vi "CreateNewProperty.vi"(5 "Physical Channels Array":string[](array[string]), 6 "JSON Text In":string, 7 "Properties Array":string[](array[string]), 8 "error IO":errorcluster, 9 "User Input":T12, 10 "Position Index":T1, 11 "Data":T2) -> (0 "error out":errorcluster, 2 "JSON Text Out":string, 3 "Data Out":T2)   [LabVIEW 2017]
uses:
  Ctrl/UserInput.ctl
  Ctrl/Data.ctl
  Ctrl/Caps.ctl
  Ctrl/Property.ctl
  Ctrl/PhysicalChannel.ctl
  Ctrl/Register.ctl
  Ctrl/Bitfield.ctl
  Ctrl/Scale.ctl
  Ctrl/ScaleType.ctl
  Ctrl/Enum.ctl
  Ctrl/EnumValue.ctl
  a49f2b7a-a89a-493e-b672-83a64a1dc848.vi
  b7239d0f-a886-4cdc-b9e9-eaf961555556.vi
  9a8c8dea-2cdf-4e02-b2f8-f2feb6ef9a15.vi
  ea6883c3-21c4-4fa9-9e68-a5003e32a3fd.vi
  c685517d-3b86-4edc-b318-7cf002de9467.vi
  83024576-e123-423a-a292-784f9ca3acef.vi
  5d470e54-f309-4a2d-b700-b5160160c7a0.vi
  2d628e2e-8e77-4fc1-a05a-5f0eb3d140a3.vi
  3a93f355-f44d-43be-885c-c8174923e2df.vi
  69acab33-e041-4299-87fe-07d24066ef73.vi
  f5ba869a-ac95-4e4c-86ff-dad057e8b940.vi
  a7fe37d0-f046-4b52-bd49-58630115636d.vi
  21b13566-51c8-4b08-b7be-3dce8c990445.vi
  f01481eb-adc2-4292-a7dc-d6c3eaadea6e.vi
  0f458bcc-7b61-44ae-a900-99c499cd9c3b.vi
  c10375a5-0795-48be-8fad-3286e309e908.vi
  5c14b599-8786-4955-9b75-2db17ef63de3.vi
  6e15b919-6c59-4ef2-a7c0-28ece143eb9f.vi
  7c4f7e53-dbd1-4e39-b078-caddc5d3bffd.vi
  11ea50df-9018-48f0-836e-47b654efc2ff.vi
  0e1caf04-e2e9-4b70-9720-e1a210467dd4.vi
  d58aa79e-fb29-4d7b-acaf-7e78ee01c68a.vi
  24b307f7-ae9b-4334-a273-07ddeeb49d19.vi
  49acb1fb-1d23-4d16-8d65-d3f60ea831e1.vi
  6c8c26da-812b-44f4-8a47-b287122740a3.vi
  6e470968-faeb-473e-94d4-9f473792bd2a.vi
  576f94e5-2af0-4523-a9f0-3304e6cbc8c1.vi
  7c2c566b-f820-4e15-b4ed-1f65cd12d5f0.vi
  0f012f77-c120-4dc7-a671-207e81cb5f49.vi
  25a589fe-9d62-4a78-be02-6bcfab6bb56e.vi
  f3b9646e-74a6-4e13-b3dc-42ccebcfd1e8.vi
  d27e821d-89cf-46bb-b5e1-9624ca9468fb.vi
  6a42c134-5544-4b97-a994-3a894c6fd8c5.vi
  628c06dd-8667-4172-93bf-cd1d4ad4abe0.vi
  4fb511c2-f303-4d71-abd1-b379f02bfd88.vi
  45fd9c47-b19a-4360-9f3e-2172322a7f8b.vi
  755fc430-c706-4afd-be3d-980f95401532.vi
  0e9b9207-256e-4707-b51c-b6ca433831fa.vi
  99d4434d-72ea-4ca1-92e2-3e4fa824596b.vi
  f10b79d4-fc05-4857-ad0d-b3836f64004d.vi
  7132fcb4-bd99-438f-a692-8292e7484c4f.vi
  cca9a672-75e7-4021-816c-68aa3c6a6872.vi
  ecd3546a-508f-424b-98fa-eb27a157b20d.vi
  0c9dfa0a-ec9d-420a-8a56-6a5b97d1e641.vi
  ccdac7b3-f8f0-4fd4-822c-79269ee8a063.vi
  3a771616-e512-457e-808b-110273b57013.vi
  d688189c-f4c5-4b6f-aec2-5bfb8a1bf2cd.vi
  ac0dcac6-9883-45e7-93cd-88fffc2866e0.vi
  3376c375-25a1-4c34-bd38-a19c28cb765e.vi
  7a403b02-5ffc-42e7-baa3-b7a4eeba28ce.vi
  01b9138b-76a2-4359-acf3-d9de97d059d9.vi
  a141bb58-9ba5-441b-868f-21200b55c099.vi
  80822c65-4f16-4974-bc2c-80759235b62b.vi
  6f6ebfe9-c60c-414d-8b12-ba3bdeeaba59.vi
  a52452e6-86e2-4211-9ca9-267b4c83b3c9.vi
  dbfa2163-7e2d-4f30-9237-4ef7c0592618.vi
  91ed7ecc-eecc-4599-94e1-676a613ecbb1.vi
  ae2bc896-6ce6-4903-bc84-87fefb09e09c.vi
  113ba1ce-32d2-48ad-819e-36eabf9c747b.vi
  4d7999a1-46fe-4a82-956d-b90eb1783e73.vi
  fd5b9c13-e0cd-4f6e-a59d-9b48d1913b00.vi
  bf6c18ca-27a2-471c-8ef5-1202f5916418.vi
  8917d4d8-2e68-438d-a95d-91d892a45299.vi
  37f20183-cbb6-408d-bc9b-499ea9cc8cf1.vi
  17a8dd43-fc52-448d-8aba-334e99b77679.vi
  8211e012-3519-4404-b0b3-339e76ea4bc1.vi
  509dba11-f6b1-40d4-b7e2-c91f78e09c4c.vi
  3b6dfc74-68ce-41c5-8a3c-09f3ccd4e9e6.vi
  556964bf-9fb0-437c-b57b-6005a56280ca.vi
  c644abda-56b7-4dd7-8add-f8f48cdb8744.vi
  9f73811a-95bf-4eb4-a8fa-f38c92d15f78.vi
  bb4007d4-f8f0-4bc5-9028-5f1cf2c35148.vi
  4f7d9488-ab40-4515-a693-da524a43faec.vi
  eddbc0d9-62dd-400d-aae9-2a28a5c77658.vi
  f57e54e9-0c83-4c4f-85ea-985bd06e531a.vi
  6f79dc5f-b950-4598-84a2-cd13e182a849.vi
  61c115c5-33ef-4a3e-bc4e-0e2805e03db5.vi
  4019a736-0945-4c3d-9530-64ae120c8d82.vi
  fc220763-ec92-4a82-8c98-1888f306469b.vi
  81716be8-6f03-4c12-be78-44b8fbb8dac1.vi
  b447dfd2-34a3-4ef0-b1a0-0449a08cdddb.vi
  0c062650-fd43-4944-b945-f8cbdc6d9a08.vi
  bc4388ac-6fed-49ed-999e-9d9af0d36177.vi
  213fb9c5-0553-47a7-8513-261bde567b61.vi
  45dea8f4-95f3-403e-9396-3338e63b5c58.vi
  198f9814-5678-407e-905c-3dffdfeb1b1a.vi
  0b3e7f97-d846-4561-b743-4d2b63a05b0c.vi
  2ce1d167-041f-4eb0-a5ff-a6bbcfc02b33.vi
  d4f37732-829b-439f-949d-15773a71446b.vi
  c2cabc7c-6f3f-4e97-9c76-69ff8817e041.vi
  a0bcf8de-4f7f-4748-830e-4ca73a3cdba5.vi
  108ef926-3dca-4005-a0d1-c4fff904fb71.vi
  decae038-41de-45d0-9a85-a35aff0e32d8.vi
  232f2805-0da1-4bd2-964f-a5a57d1a0789.vi
  b481430d-8ad2-4f6e-8535-813648ab6332.vi
  30ebd30d-697e-41d4-a062-6538e9b0372d.vi
  3e2a4e09-f947-4d87-9f6b-36e026663a87.vi
  4de69aee-0985-453e-b62a-95ac3040a333.vi
  a82c2a40-5500-42ec-81fe-51a317ee7e6a.vi
  4ea25b15-c434-4186-b702-6004432441e7.vi
  1f846b06-a524-4db4-a3bc-67689fb64464.vi
  8cc0f9d5-1403-42f5-8db9-98bc4be2fcad.vi
  e01775d1-2ca2-49e0-b186-643bd2c40956.vi
  203d3e81-1240-40e6-b528-fe3fc3fb6b71.vi
  b90cfbf0-b34a-4f7c-a92c-1bf1608e7875.vi
  17010cc0-3e9d-4f94-9fb8-6f8c3e52e337.vi
  31c470be-9090-43e5-9e9c-e90aeaef58ff.vi
  65070d91-edea-43b9-8fa4-4e2d47d23c2a.vi
  223cc870-c1bd-4fed-9a4e-cb6bbe7d487d.vi
  231ecd50-a15c-4ed1-a0c9-2424d186b4de.vi
  36281ff1-d9a9-4575-bd1c-3efb6e2311e5.vi
  624e145d-2cd7-4bd9-b329-75a63af49bab.vi
  cfc68e07-b182-4d06-a56e-000b2c92bce0.vi
  0a8ea711-960b-4203-93a6-dad2a0ce5ccf.vi
  27813dee-b6cf-4adb-b65a-f979060e7e79.vi
  1f1b6db9-9b07-4b01-9a35-2055f5be4eb1.vi
  ace04026-a7e6-4f2f-b899-111909789ab4.vi
  37535dc1-fec1-4151-9bd0-9935b704efa5.vi
  db3b4f8a-2deb-4574-ad41-4f9ae64a690f.vi
  6e899c75-a155-4662-bc59-3d9896a22a99.vi
  f9819b1f-b189-4309-8c14-53bc3d75f35f.vi
  6878b97e-9808-4441-b6cb-f4989035cf89.vi
  40b71344-1fb3-4cdd-a6ad-9b0b64e136ec.vi
  9c3c6458-e941-4b27-8d55-2b4a0fd28597.vi
  39623eaf-85e6-4175-8452-6887610aa769.vi
  1149246f-1cb2-4460-baf6-518fc77c3398.vi
  94badf7b-9ba4-4923-94d3-547b74146f8e.vi
  ffb6c1ad-0599-4325-8e09-657e99a7831d.vi
  51fd1ea7-ce8f-4a70-a74f-9fc830ed3e6b.vi
  de89801e-8830-4ce5-860e-6e3e2d97c53c.vi
  455b00cc-8d48-4a28-be52-9894321e9b13.vi
  9e4596ea-b512-429e-ae0e-35bad6f11e4a.vi
  d6d440e2-9f68-4db2-b22d-75274f54af10.vi
  1256f0d8-c1ca-45fc-a187-c743900cc4a2.vi
  9439dccc-9f4c-481b-bf63-cbedd9744780.vi
  1f2e0b96-ad1d-4f53-bf6b-c3e13ad15049.vi
  4cd03f52-d737-4399-b5f9-45d06f489655.vi
  14ebd26c-c7b1-4e24-86d1-22f775b8f9ab.vi
  8a9c42ea-46d3-4fe9-9435-a8b3a4a2dbd4.vi
  3a6543c7-dfa5-4b63-b6d3-167b518bbb5e.vi
  5a92ceff-b602-480b-bb39-7b08cb863a45.vi
  d378d0bf-cb50-4329-b507-76bc9876ca06.vi
  7e87eee9-c7ed-45a5-bcca-739a3caf24b9.vi
  f2f04b58-7349-4c1d-a7d6-26891e21feea.vi
  bf4bca74-9d66-4959-9a8b-143b177785cd.vi
  04733de7-f337-4faf-8c84-b7833aa6f2cb.vi
  74f378fe-b6f6-4528-9979-942041c20273.vi
  c32d4527-d702-4456-8891-4932f3849ab6.vi
  74301831-9c69-485b-8e5c-16671aac40f0.vi
  32197667-d662-404d-af3b-3c9461875803.vi
  26d8f128-faf4-4dc7-be93-989510b637ce.vi
  f34d1c9c-ef35-4bff-872b-d236ed75701e.vi
  9c27fe3a-8c23-4b01-b34b-ef9b2563181d.vi
  a6395615-55d0-428c-9b5d-c0b31a22a7cf.vi
  f2764ccd-c2d5-4c9f-af8e-47687746aee1.vi
  e5379eb7-e7bb-42e7-910b-1b038f3940f8.vi
  a0e0f5c1-ff2b-49b7-a7b9-a60d0cd9baa7.vi
  a0b0d031-bf61-4b01-9fca-99c15f00df1f.vi
  54d28dfd-e1e7-45d6-aa43-71dfc314fd28.vi
  ab9abbc4-570d-4bb5-bc1a-691eeb63bc1d.vi
  d1ce7e24-64f3-4c43-ab40-66c03b4f9e3e.vi
  b237b2f1-2f83-437a-9cea-1bce77fd5025.vi
  044d47e4-0514-4989-8b3e-8a398604f3d7.vi
  c63cd178-caa2-4b18-8318-2349136bf0e1.vi
  4b639117-fa7a-4c0e-8ad7-bca49a2943c3.vi
  8267567e-f780-4e05-b009-d0c9ce0abba4.vi
  1625688c-520d-43a3-ab9a-e66d702972f2.vi
  44449f3f-58ce-45d9-97d0-2b38db85702a.vi
  f909daa1-f824-43b3-83b3-b8b77778ee66.vi
  a97c2141-69b1-4da5-94ca-ebac57d47087.vi
  b0e5809b-780b-4791-a098-08ecc8fea483.vi
  3022a1d8-e834-49f8-aa3d-1b2c8a074b58.vi
  a74e2ca7-2cff-4482-b120-7da61f7f9ad3.vi
  e2416475-e97a-4f09-a291-685253a7cfe7.vi
  313abf92-0b2c-41a6-89ad-da4ba565ce18.vi
  37aa6e6a-6e49-48fc-97e0-4a9a28f52783.vi
  42e813b3-8dc3-471a-9ba1-21131290105b.vi
  6f02c78c-2bb0-4da4-870c-847981bce678.vi
  006840be-01be-4ebd-9b8f-ea77a6ba57aa.vi
  83ec3a63-defe-4e3b-a6ed-e0f6b07438b7.vi
  76608141-6b6b-44ec-b072-9a8bd16893bc.vi
  661c9a8c-c5b5-406e-a622-3d4232183939.vi
  448871fc-56c7-4969-ae73-d107eae8dd61.vi
  67a8e6fe-4925-4bd0-bf84-9d9d2ff2a511.vi
  e0e6f61b-f592-4636-85da-145c07327336.vi
  05b159be-fb2d-4452-84c3-9ba3097d799d.vi
  66a5adf1-5026-465b-8117-59515cd5681b.vi
  89332561-ea55-4d6a-8c47-78ecf90b24dc.vi
  42cf89a1-8e03-4f53-8d52-799e9435a61c.vi
  96527726-a160-4a48-adef-fe795eb6a5ca.vi
  36013bd7-b93e-491b-a104-af11587fd964.vi
  f1628db2-2072-415f-964c-f240b5113352.vi
  6395648c-62af-41db-b829-02cd2fba18d1.vi
  0d4c42cd-1dc5-4f20-868b-863dbe6493db.vi
  454f590e-240f-4e40-8cf2-0be346249117.vi
  eca76937-d954-4f66-b29c-5125c898f574.vi
  ee8ef92e-b5c6-4b6c-9e99-f238648b3acd.vi
  ab44ab14-7959-48f0-b172-dac530811317.vi
  fe65aa24-0d15-4b88-8a81-a6b00e8cc108.vi
  47278b13-07ad-44b4-92ee-55cb8c7775f7.vi
  32afd39a-e2cc-43d6-8b91-cc3721be6205.vi
  72a5a9e2-8cc7-4781-b6ce-fe396b598b40.vi
  aa930b89-a957-4a40-aea5-f072bec8f2e0.vi
  ae0460c2-7f2e-440b-b89e-9afba5751a8a.vi
  d2cfe406-efaa-4813-911a-e8cc1010b633.vi
  53ced5e1-6cfb-4c56-ae99-55efe528f378.vi
  2e78f98a-ab78-448d-8ebd-4acd63531133.vi
  88442ee8-73f3-4212-ac74-ab778edeacb7.vi
  1332a019-3d0f-4c16-8ae1-7ee48909245a.vi
  df3c917c-2193-40a5-ba35-6d5d70650e51.vi
  edce4bd0-27e9-42af-8081-06bf6614b3f1.vi
  a8ec8fbb-1ef4-4c47-b821-8822cada8249.vi
  <vilib>/JDP Science/JSONtext/String Subset.vi
  <vilib>/JDP Science/JSONtext/Variant to JSON Text.vi
  <vilib>/JDP Science/JSONtext/Parsing/Parse Full Path or Item Name.vi
  <vilib>/JDP Science/JSONtext/Offset/Find Item Locations by Path.vi
  <vilib>/JDP Science/JSONtext/JSONtext.lvlib
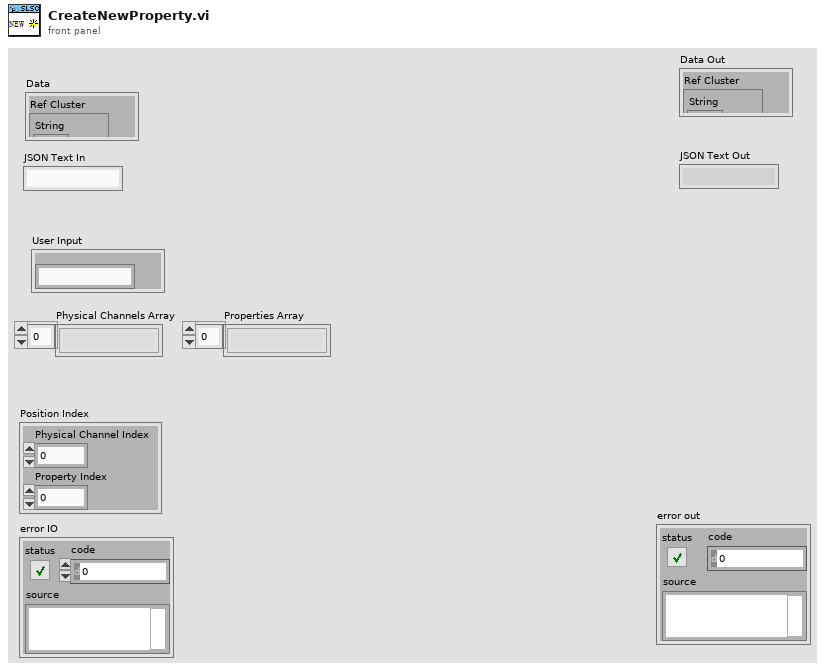
[diagram p1: front panel]
types:
  T1 = cluster{"Physical Channel Index":i32, "Property Index":i32}
  T2 = typedef "Data.ctl" = cluster{"Ref Cluster":cluster{"String":refnum<vi>, "U8":refnum<vi>, "I8":refnum<vi>, "U32":refnum<vi>, "I32":refnum<vi>, "U64":refnum<vi>, "I64":refnum<vi>, "Ring":refnum<vi>, "DBL":refnum<vi>, "Add":refnum<vi>, "Remove":refnum<vi>, "Property tree":refnum<vi>, "confirm":refnum<vi>}, "JSON Text":string, "Original JSON Text":string, "Caps":T3, "SLSC Output Tree":cluster{"Left Cell String":string, "Child Text":string[], "Child Tag":string, "Item Indent":i32, "Child Only?":bool, "Glyph Index":i32, "offline value":variant}[], "Ref Index and Control Type":cluster{"index":i32, "Datatype":string}, "Selected Type and name":cluster{"Selected Type":enum16{"Property", "Physical Channel", "Other"}, "Selected Property Name":string}, "Update whole Tree?":bool}
  T3 = typedef "Caps.ctl" = cluster{"properties":T4[], "physical channels":T5[], "registers":T6[], "scales":T8[], "enums":T10[], "productName":string}
  T4 = typedef "Property.ctl" = cluster{"name":string, "bitfield":string, "value":variant, "dataType":string, "min":variant, "max":variant, "scale":string, "access":string}
  T5 = typedef "PhysicalChannel.ctl" = cluster{"name":string, "properties":T4[]}
  T6 = typedef "Register.ctl" = cluster{"name":string, "address":i32, "size":i32, "bitfields":T7[], "initialValue":variant, "connectedProperties":string[]}
  T7 = typedef "Bitfield.ctl" = cluster{"name":string, "offset":i32, "size":i32, "signed":bool}
  T8 = typedef "Scale.ctl" = cluster{"name":string, "type":T9, "params":variant}
  T9 = typedef "ScaleType.ctl" = enum16{"NoScale", "Table", "Polynomial", "Linear"}
  T10 = typedef "Enum.ctl" = cluster{"name":string, "values":T11[]}
  T11 = typedef "EnumValue.ctl" = cluster{"name":string, "value":i32}
  T12 = typedef "UserInput.ctl" = cluster{"NewPropertyParameter":cluster{"Name":string, "DataType":enum16{"String", "Double", "U64", "I64", "U32", "I32", "Bool"}, "Bitfield":u16, "Access":u16, "Description":string, "Documentation":string, "OK Button":bool, "Scale method":u16, "Write a Register?":bool, "Write a Range?":bool, "Value_Cluster":cluster{"DBL":dbl, "Ring":u16, "I64":i64, "U64":u64, "I32":i32, "U32":u32, "I8":i8, "U8":u8, "String":string}}, "Min_Max_Cluster":cluster{"Min(Double)":dbl, "Max(Double)":dbl, "Min(U64)":u64, "Max(U64)":u64, "Min(I64)":i64, "Max(I64)":i64, "Min(U32)":u32, "Max(U32)":u32, "Min(I32)":i32, "Max(I32)":i32}, "Scale method":string, "Access":string, "Bitfield":string}
  T13 = enum16{"String", "Double", "U64", "I64", "U32", "I32", "Bool"}
  T14 = cluster{"DBL":dbl, "Ring":u16, "I64":i64, "U64":u64, "I32":i32, "U32":u32, "I8":i8, "U8":u8, "String":string}
  T15 = cluster{"Min(Double)":dbl, "Max(Double)":dbl, "Min(U64)":u64, "Max(U64)":u64, "Min(I64)":i64, "Max(I64)":i64, "Min(U32)":u32, "Max(U32)":u32, "Min(I32)":i32, "Max(I32)":i32}
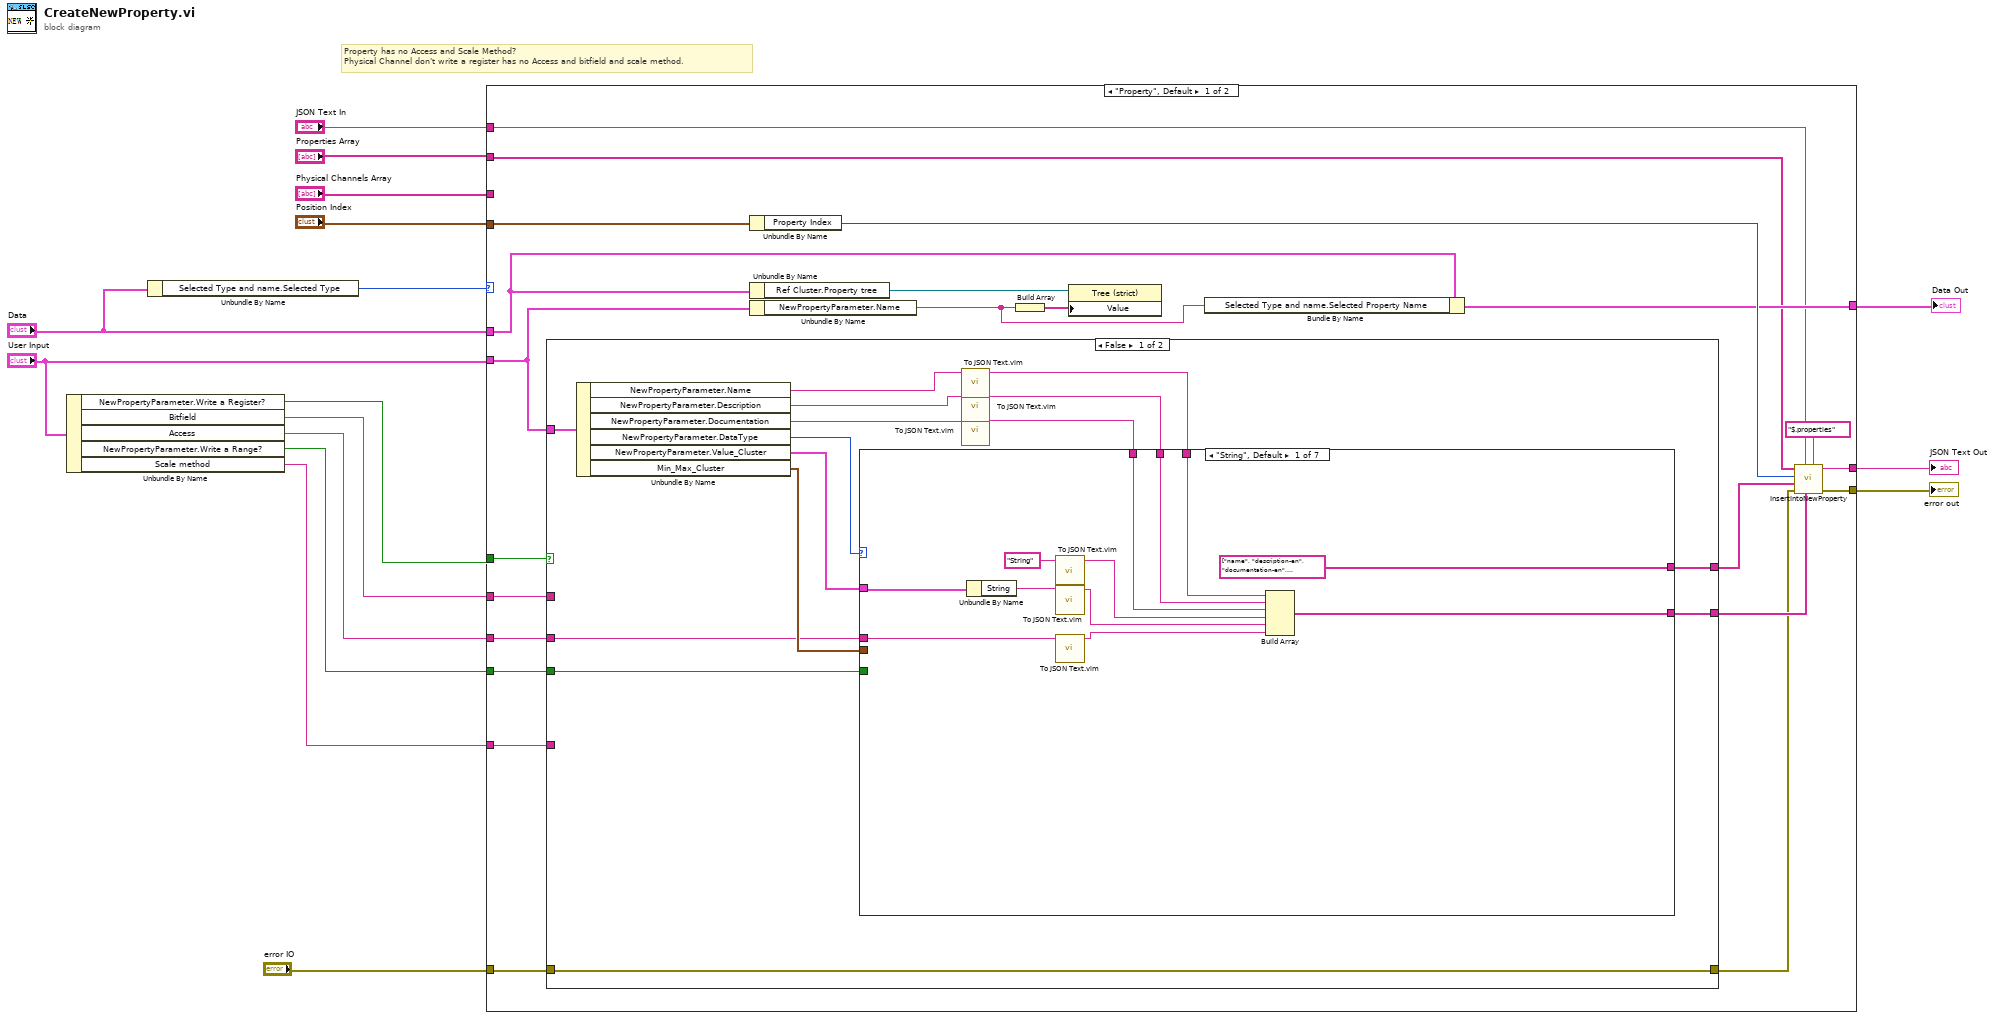
[diagram p0: block diagram]
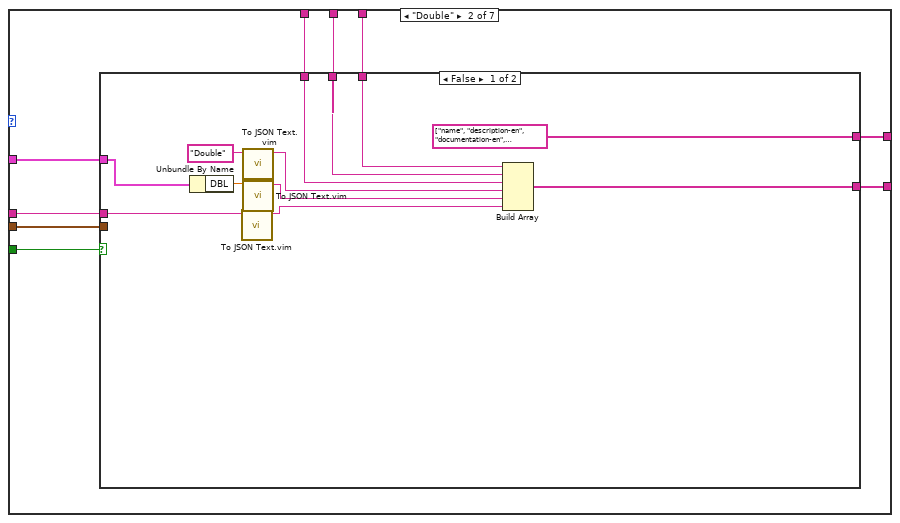
[diagram p2: hidden frame]
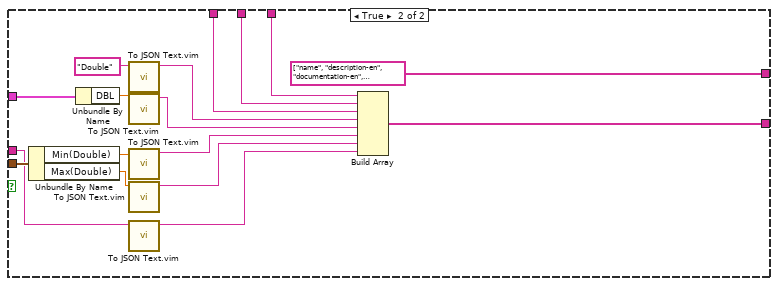
[diagram p3: hidden frame]
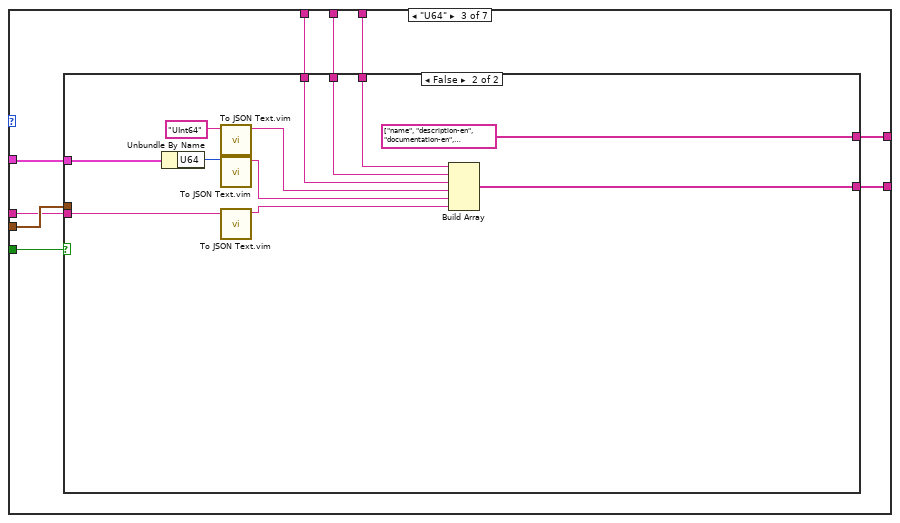
[diagram p4: hidden frame]
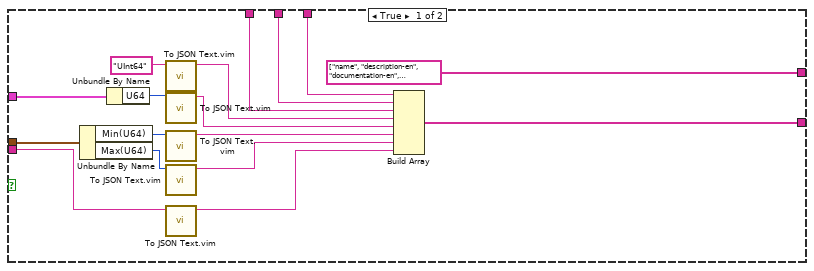
[diagram p5: hidden frame]
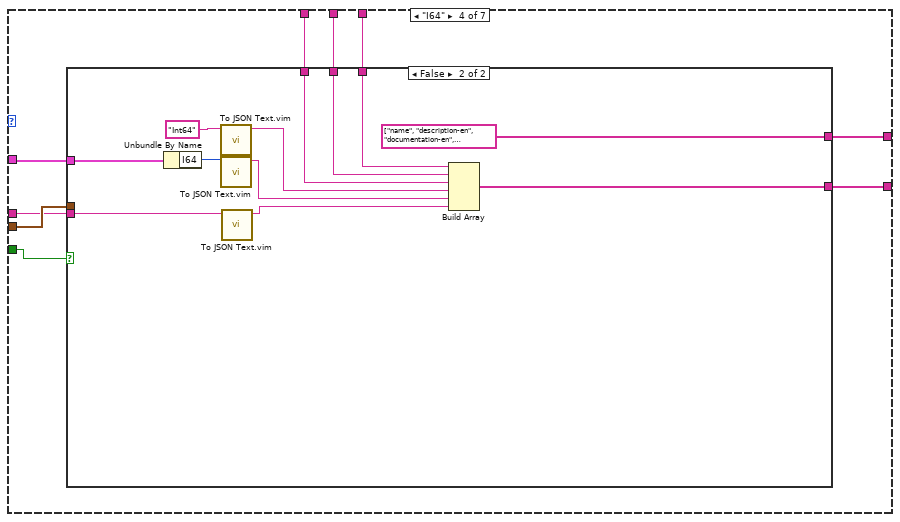
[diagram p6: hidden frame]
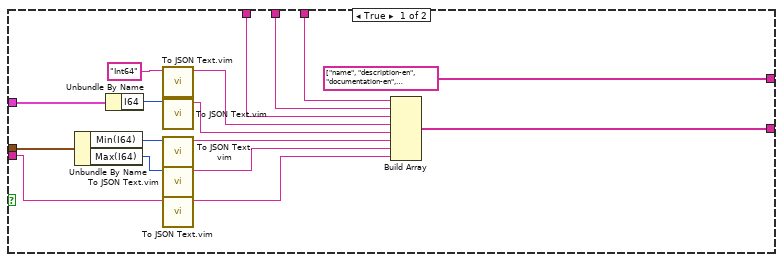
[diagram p7: hidden frame]
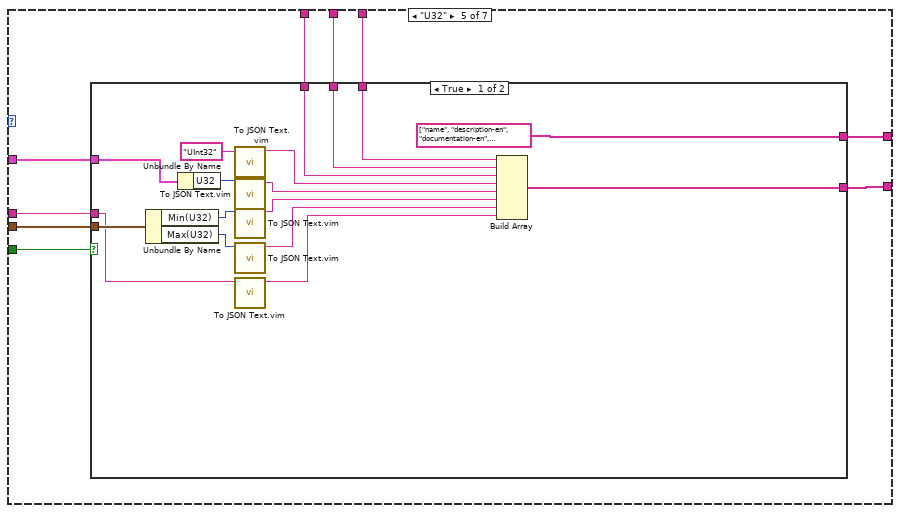
[diagram p8: hidden frame]
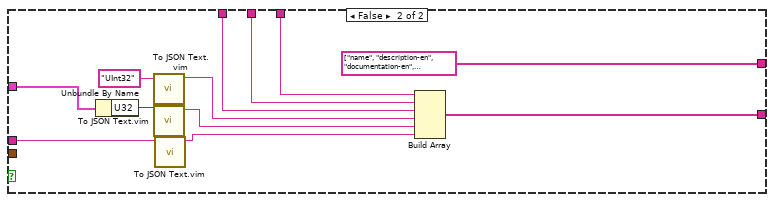
[diagram p9: hidden frame]
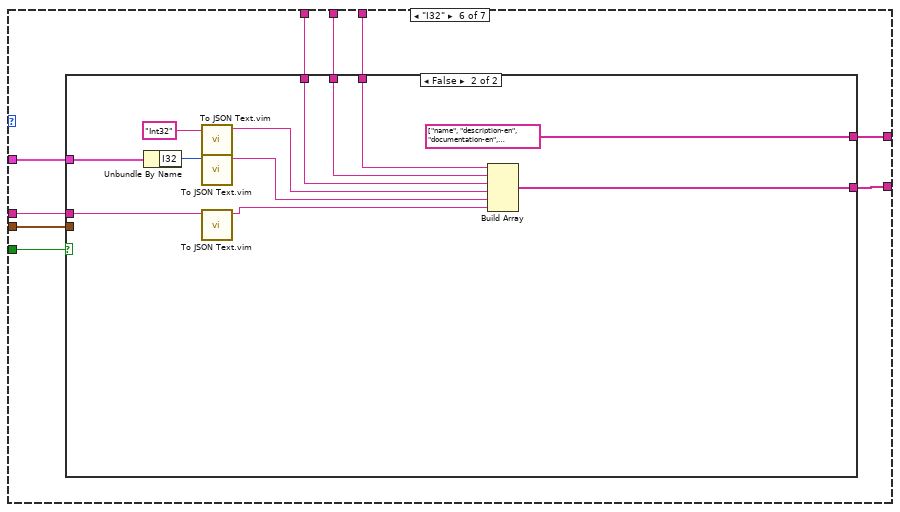
[diagram p10: hidden frame]
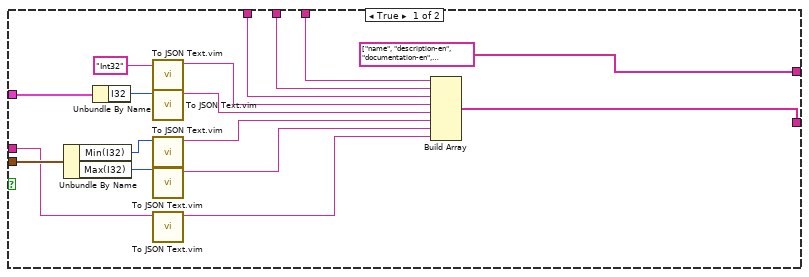
[diagram p11: hidden frame]
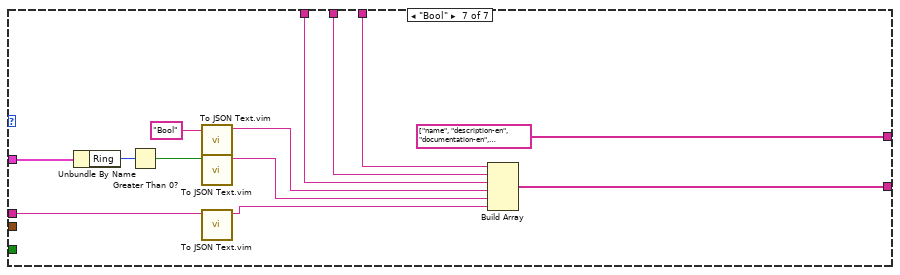
[diagram p12: hidden frame]
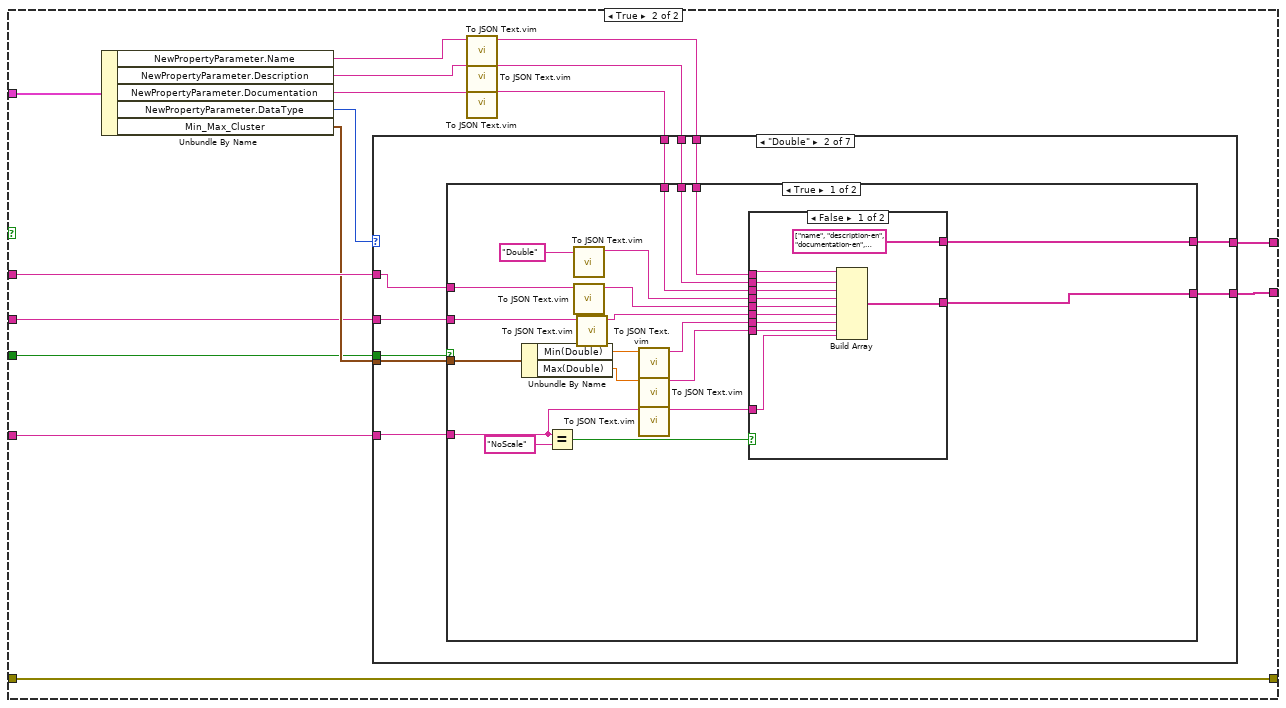
[diagram p13: hidden frame]
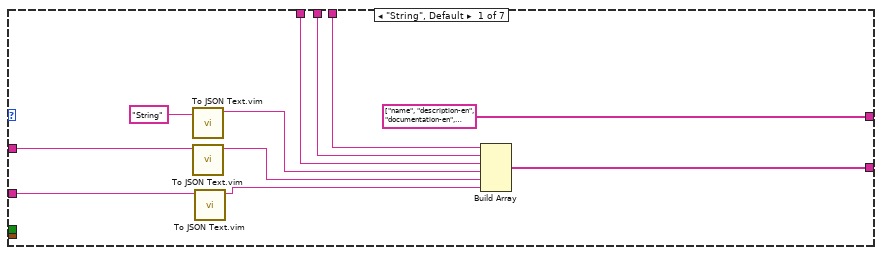
[diagram p14: hidden frame]
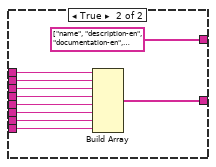
[diagram p15: hidden frame]
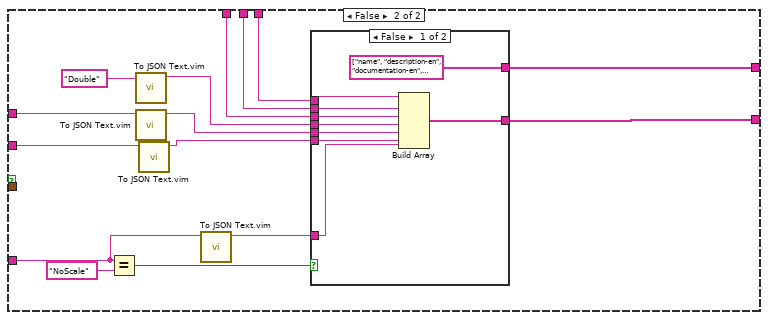
[diagram p16: hidden frame]
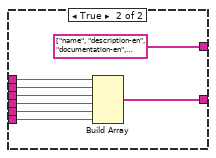
[diagram p17: hidden frame]
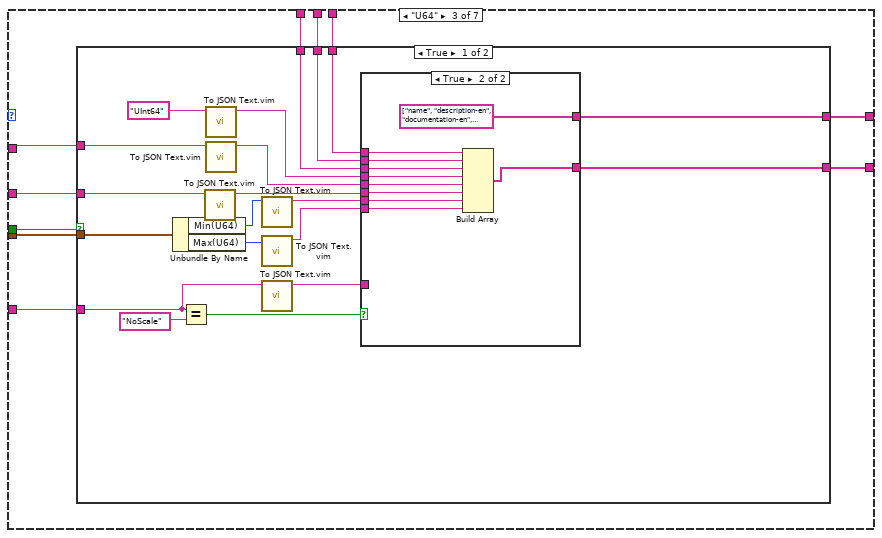
[diagram p18: hidden frame]
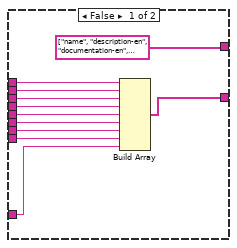
[diagram p19: hidden frame]
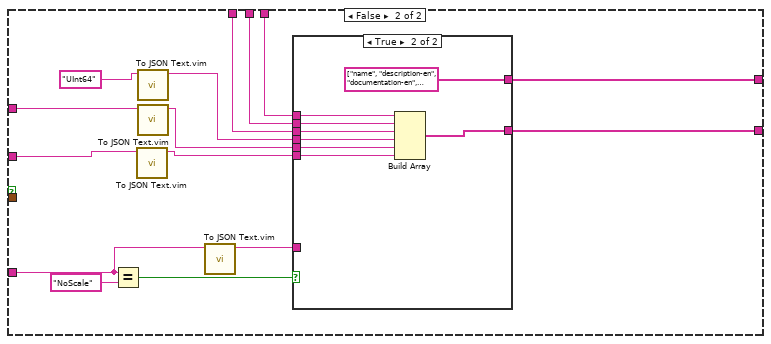
[diagram p20: hidden frame]
diagram:
  # "Property has no Access and Scale Method?\nPhysical Channel don't write a register has no Access and bitfield and scale method."
  n1 = Unbundle By Name("User Input") -> ("NewPropertyParameter.Write a Register?"=w7:bool, "Bitfield"=w6:string, "Access"=w5:string, "NewPropertyParameter.Write a Range?"=w4:bool, "Scale method"=w3:string)
  n2 = Unbundle By Name("Data") -> ("Selected Type and name.Selected Type"=w1:enum16{"Property", "Physical Channel", "Other"})
  n3 = case shown="\"Property\", Default" w1 {
    tunnel: w7 -> [w38 w754]
    tunnel: "error IO" -> [w37 w728]
    tunnel: "Properties Array" -> [w20 _]
    tunnel: "JSON Text In" -> [w23 w731]
    tunnel: [w19 w730] -> w10
    tunnel: [w18 w729] -> w9
    tunnel: w6 -> [w36 w753]
    tunnel: w5 -> [w35 w752]
    tunnel: "Physical Channels Array" -> [_ w747]
    tunnel: "User Input" -> [w30 w743]
    tunnel: "Position Index" -> [w34 w749]
    tunnel: w3 -> [w32 w745]
    tunnel: w4 -> [w31 w744]
    tunnel: "Data" -> [w27 w740]
    tunnel: [w25 w739] -> w11
    frame "Property", Default {
      n4 = case shown="False" w38 {
        tunnel: w37 -> [w44 w272]
        tunnel: w36 -> [_ w277]
        tunnel: w35 -> [w39 w275]
        tunnel: [w46 w274] -> w22
        tunnel: [w45 w273] -> w21
        tunnel: [w44 w272] -> w17
        tunnel: w30 -> [w43 w271]
        tunnel: w32 -> [_ w270]
        tunnel: w31 -> [w40 w269]
        frame False {
          n5 = Unbundle By Name(w43) -> ("NewPropertyParameter.Name"=w53:string, "NewPropertyParameter.Description"=w52:string, "NewPropertyParameter.Documentation"=w51:string, "NewPropertyParameter.DataType"=w50:T13, "NewPropertyParameter.Value_Cluster"=w42:T14, "Min_Max_Cluster"=w41:T15)
          n6 = call "To JSON Text.vim"("Anything"=w53) -> ("<JSON>"=w49:string)  [unwired: 9 in, 1 out]
          n7 = call "To JSON Text.vim"("Anything"=w52) -> ("<JSON>"=w48:string)  [unwired: 9 in, 1 out]
          n8 = call "To JSON Text.vim"("Anything"=w51) -> ("<JSON>"=w47:string)  [unwired: 9 in, 1 out]
          n9 = case shown="\"String\", Default" w50 {
            tunnel: w42 -> [w65 w74 w112 w150 w184 w222 w264]
            tunnel: w49 -> [w61 w73 w111 w149 w187 w225 w267]
            tunnel: w48 -> [w60 w72 w110 w148 w186 w224 w266]
            tunnel: w47 -> [w59 w71 w109 w147 w185 w223 w265]
            tunnel: [string[] ["name", "description-en", "documentation-en", "dataType", "value", "access"] ("Item Names") w69 w107 w145 w188 w226 string[] ["name", "description-en", "documentation-en", "dataType", "value", "access"] ("Item Names")] -> w46
            tunnel: [w56 w70 w108 w146 w182 w220 w263] -> w45
            tunnel: w41 -> [_ w68 w106 w144 w183 w221 _]
            tunnel: w40 -> [_ w67 w105 w143 w181 w219 _]
            tunnel: w39 -> [w55 w66 w104 w142 w180 w218 w257]
            frame "String", Default {
              n10 = Unbundle By Name(w65) -> ("String"=w64:string)
              n11 = call "To JSON Text.vim"("Anything"="String") -> ("<JSON>"=w58:string)  [unwired: 9 in, 1 out]
              n12 = call "To JSON Text.vim"("Anything"=w64) -> ("<JSON>"=w57:string)  [unwired: 9 in, 1 out]
              n13 = call "To JSON Text.vim"("Anything"=w55) -> ("<JSON>"=w54:string)  [unwired: 9 in, 1 out]
              n14 = Build Array(w61, w60, w59, w58, w57, w54) -> (w56:string[])
            }
            frame "Double" {
              n15 = case shown="False" w67 {
                tunnel: w74 -> [w82 w103]
                tunnel: w73 -> [w81 w100]
                tunnel: w72 -> [w80 w99]
                tunnel: w71 -> [w79 w98]
                tunnel: [w77 w95] -> w70
                tunnel: [string[] ["name", "description-en", "documentation-en", "dataType", "value", "access"] ("Item Names") string[] ["name", "description-en", "documentation-en", "dataType", "value", "min", "max", "access"] ("Item Names")] -> w69
                tunnel: w68 -> [_ w93]
                tunnel: w66 -> [w76 w88]
                frame False {
                  n16 = Unbundle By Name(w82) -> ("DBL"=w86:dbl)
                  n17 = call "To JSON Text.vim"("Anything"=w76) -> ("<JSON>"=w75:string)  [unwired: 9 in, 1 out]
                  n18 = call "To JSON Text.vim"("Anything"="Double") -> ("<JSON>"=w84:string)  [unwired: 9 in, 1 out]
                  n19 = call "To JSON Text.vim"("Anything"=w86) -> ("<JSON>"=w83:string)  [unwired: 9 in, 1 out]
                  n20 = Build Array(w81, w80, w79, w84, w83, w75) -> (w77:string[])
                }
                frame True {
                  n21 = Unbundle By Name(w93) -> ("Min(Double)"=w92:dbl, "Max(Double)"=w91:dbl)
                  n22 = Unbundle By Name(w103) -> ("DBL"=w102:dbl)
                  n23 = call "To JSON Text.vim"("Anything"="Double") -> ("<JSON>"=w97:string)  [unwired: 9 in, 1 out]
                  n24 = call "To JSON Text.vim"("Anything"=w102) -> ("<JSON>"=w96:string)  [unwired: 9 in, 1 out]
                  n25 = call "To JSON Text.vim"("Anything"=w92) -> ("<JSON>"=w90:string)  [unwired: 9 in, 1 out]
                  n26 = call "To JSON Text.vim"("Anything"=w91) -> ("<JSON>"=w89:string)  [unwired: 9 in, 1 out]
                  n27 = call "To JSON Text.vim"("Anything"=w88) -> ("<JSON>"=w87:string)  [unwired: 9 in, 1 out]
                  n28 = Build Array(w100, w99, w98, w97, w96, w90, w89, w87) -> (w95:string[])
                }
              }
            }
            frame "U64" {
              n29 = case shown="False" w105 {
                tunnel: w112 -> [w129 w141]
                tunnel: w111 -> [w126 w138]
                tunnel: w110 -> [w125 w137]
                tunnel: w109 -> [w124 w136]
                tunnel: [w121 w133] -> w108
                tunnel: [string[] ["name", "description-en", "documentation-en", "dataType", "value", "min", "max", "access"] ("Item Names") string[] ["name", "description-en", "documentation-en", "dataType", "value", "access"] ("Item Names")] -> w107
                tunnel: w106 -> [w119 _]
                tunnel: w104 -> [w114 w131]
                frame True {
                  n30 = Unbundle By Name(w119) -> ("Min(U64)"=w118:u64, "Max(U64)"=w117:u64)
                  n31 = Unbundle By Name(w129) -> ("U64"=w128:u64)
                  n32 = call "To JSON Text.vim"("Anything"="UInt64") -> ("<JSON>"=w123:string)  [unwired: 9 in, 1 out]
                  n33 = call "To JSON Text.vim"("Anything"=w128) -> ("<JSON>"=w122:string)  [unwired: 9 in, 1 out]
                  n34 = call "To JSON Text.vim"("Anything"=w118) -> ("<JSON>"=w116:string)  [unwired: 9 in, 1 out]
                  n35 = call "To JSON Text.vim"("Anything"=w117) -> ("<JSON>"=w115:string)  [unwired: 9 in, 1 out]
                  n36 = call "To JSON Text.vim"("Anything"=w114) -> ("<JSON>"=w113:string)  [unwired: 9 in, 1 out]
                  n37 = Build Array(w126, w125, w124, w123, w122, w116, w115, w113) -> (w121:string[])
                }
                frame False {
                  n38 = Unbundle By Name(w141) -> ("U64"=w140:u64)
                  n39 = call "To JSON Text.vim"("Anything"="UInt64") -> ("<JSON>"=w135:string)  [unwired: 9 in, 1 out]
                  n40 = call "To JSON Text.vim"("Anything"=w140) -> ("<JSON>"=w134:string)  [unwired: 9 in, 1 out]
                  n41 = call "To JSON Text.vim"("Anything"=w131) -> ("<JSON>"=w130:string)  [unwired: 9 in, 1 out]
                  n42 = Build Array(w138, w137, w136, w135, w134, w130) -> (w133:string[])
                }
              }
            }
            frame "I64" {
              n43 = case shown="False" w143 {
                tunnel: w150 -> [w167 w179]
                tunnel: w149 -> [w164 w176]
                tunnel: w148 -> [w163 w175]
                tunnel: w147 -> [w162 w174]
                tunnel: [w159 w171] -> w146
                tunnel: [string[] ["name", "description-en", "documentation-en", "dataType", "value", "min", "max", "access"] ("Item Names") string[] ["name", "description-en", "documentation-en", "dataType", "value", "access"] ("Item Names")] -> w145
                tunnel: w144 -> [w157 _]
                tunnel: w142 -> [w152 w169]
                frame True {
                  n44 = Unbundle By Name(w157) -> ("Min(I64)"=w156:i64, "Max(I64)"=w155:i64)
                  n45 = Unbundle By Name(w167) -> ("I64"=w166:i64)
                  n46 = call "To JSON Text.vim"("Anything"="Int64") -> ("<JSON>"=w161:string)  [unwired: 9 in, 1 out]
                  n47 = call "To JSON Text.vim"("Anything"=w166) -> ("<JSON>"=w160:string)  [unwired: 9 in, 1 out]
                  n48 = call "To JSON Text.vim"("Anything"=w156) -> ("<JSON>"=w154:string)  [unwired: 9 in, 1 out]
                  n49 = call "To JSON Text.vim"("Anything"=w155) -> ("<JSON>"=w153:string)  [unwired: 9 in, 1 out]
                  n50 = call "To JSON Text.vim"("Anything"=w152) -> ("<JSON>"=w151:string)  [unwired: 9 in, 1 out]
                  n51 = Build Array(w164, w163, w162, w161, w160, w154, w153, w151) -> (w159:string[])
                }
                frame False {
                  n52 = Unbundle By Name(w179) -> ("I64"=w178:i64)
                  n53 = call "To JSON Text.vim"("Anything"="Int64") -> ("<JSON>"=w173:string)  [unwired: 9 in, 1 out]
                  n54 = call "To JSON Text.vim"("Anything"=w178) -> ("<JSON>"=w172:string)  [unwired: 9 in, 1 out]
                  n55 = call "To JSON Text.vim"("Anything"=w169) -> ("<JSON>"=w168:string)  [unwired: 9 in, 1 out]
                  n56 = Build Array(w176, w175, w174, w173, w172, w168) -> (w171:string[])
                }
              }
            }
            frame "U32" {
              n57 = case shown="True" w181 {
                tunnel: [string[] ["name", "description-en", "documentation-en", "dataType", "value", "min", "max", "access"] ("Item Names") string[] ["name", "description-en", "documentation-en", "dataType", "value", "access"] ("Item Names")] -> w188
                tunnel: w187 -> [w204 w216]
                tunnel: w186 -> [w203 w215]
                tunnel: w185 -> [w202 w214]
                tunnel: w184 -> [w199 w211]
                tunnel: w183 -> [w198 _]
                tunnel: [w191 w208] -> w182
                tunnel: w180 -> [w190 w207]
                frame True {
                  n58 = Unbundle By Name(w198) -> ("Min(U32)"=w197:u32, "Max(U32)"=w196:u32)
                  n59 = Unbundle By Name(w199) -> ("U32"=w200:u32)
                  n60 = call "To JSON Text.vim"("Anything"="UInt32") -> ("<JSON>"=w195:string)  [unwired: 9 in, 1 out]
                  n61 = call "To JSON Text.vim"("Anything"=w200) -> ("<JSON>"=w194:string)  [unwired: 9 in, 1 out]
                  n62 = call "To JSON Text.vim"("Anything"=w197) -> ("<JSON>"=w193:string)  [unwired: 9 in, 1 out]
                  n63 = call "To JSON Text.vim"("Anything"=w196) -> ("<JSON>"=w192:string)  [unwired: 9 in, 1 out]
                  n64 = call "To JSON Text.vim"("Anything"=w190) -> ("<JSON>"=w189:string)  [unwired: 9 in, 1 out]
                  n65 = Build Array(w204, w203, w202, w195, w194, w193, w192, w189) -> (w191:string[])
                }
                frame False {
                  n66 = Unbundle By Name(w211) -> ("U32"=w212:u32)
                  n67 = call "To JSON Text.vim"("Anything"="UInt32") -> ("<JSON>"=w210:string)  [unwired: 9 in, 1 out]
                  n68 = call "To JSON Text.vim"("Anything"=w212) -> ("<JSON>"=w209:string)  [unwired: 9 in, 1 out]
                  n69 = call "To JSON Text.vim"("Anything"=w207) -> ("<JSON>"=w206:string)  [unwired: 9 in, 1 out]
                  n70 = Build Array(w216, w215, w214, w210, w209, w206) -> (w208:string[])
                }
              }
            }
            frame "I32" {
              n71 = case shown="False" w219 {
                tunnel: [string[] ["name", "description-en", "documentation-en", "dataType", "value", "min", "max", "access"] ("Item Names") string[] ["name", "description-en", "documentation-en", "dataType", "value", "access"] ("Item Names")] -> w226
                tunnel: w225 -> [w242 w254]
                tunnel: w224 -> [w241 w253]
                tunnel: w223 -> [w240 w252]
                tunnel: w222 -> [w238 w250]
                tunnel: w221 -> [w236 _]
                tunnel: [w229 w246] -> w220
                tunnel: w218 -> [w228 w245]
                frame True {
                  n72 = Unbundle By Name(w236) -> ("Min(I32)"=w233:i32, "Max(I32)"=w232:i32)
                  n73 = Unbundle By Name(w238) -> ("I32"=w237:i32)
                  n74 = call "To JSON Text.vim"("Anything"="Int32") -> ("<JSON>"=w235:string)  [unwired: 9 in, 1 out]
                  n75 = call "To JSON Text.vim"("Anything"=w237) -> ("<JSON>"=w234:string)  [unwired: 9 in, 1 out]
                  n76 = call "To JSON Text.vim"("Anything"=w233) -> ("<JSON>"=w231:string)  [unwired: 9 in, 1 out]
                  n77 = call "To JSON Text.vim"("Anything"=w232) -> ("<JSON>"=w230:string)  [unwired: 9 in, 1 out]
                  n78 = call "To JSON Text.vim"("Anything"=w228) -> ("<JSON>"=w227:string)  [unwired: 9 in, 1 out]
                  n79 = Build Array(w242, w241, w240, w235, w234, w231, w230, w227) -> (w229:string[])
                }
                frame False {
                  n80 = Unbundle By Name(w250) -> ("I32"=w249:i32)
                  n81 = call "To JSON Text.vim"("Anything"="Int32") -> ("<JSON>"=w248:string)  [unwired: 9 in, 1 out]
                  n82 = call "To JSON Text.vim"("Anything"=w249) -> ("<JSON>"=w247:string)  [unwired: 9 in, 1 out]
                  n83 = call "To JSON Text.vim"("Anything"=w245) -> ("<JSON>"=w244:string)  [unwired: 9 in, 1 out]
                  n84 = Build Array(w254, w253, w252, w248, w247, w244) -> (w246:string[])
                }
              }
            }
            frame "Bool" {
              n85 = Unbundle By Name(w264) -> ("Ring"=w261:u16)
              n86 = Greater Than 0?(x=w261) -> (x > 0?=w258:bool)
              n87 = call "To JSON Text.vim"("Anything"="Bool") -> ("<JSON>"=w260:string)  [unwired: 9 in, 1 out]
              n88 = call "To JSON Text.vim"("Anything"=w258) -> ("<JSON>"=w259:string)  [unwired: 9 in, 1 out]
              n89 = call "To JSON Text.vim"("Anything"=w257) -> ("<JSON>"=w256:string)  [unwired: 9 in, 1 out]
              n90 = Build Array(w267, w266, w265, w260, w259, w256) -> (w263:string[])
            }
          }
        }
        frame True {
          n91 = Unbundle By Name(w271) -> ("NewPropertyParameter.Name"=w284:string, "NewPropertyParameter.Description"=w283:string, "NewPropertyParameter.Documentation"=w282:string, "NewPropertyParameter.DataType"=w281:T13, "Min_Max_Cluster"=w276:T15)
          n92 = call "To JSON Text.vim"("Anything"=w284) -> ("<JSON>"=w280:string)  [unwired: 9 in, 1 out]
          n93 = call "To JSON Text.vim"("Anything"=w283) -> ("<JSON>"=w279:string)  [unwired: 9 in, 1 out]
          n94 = call "To JSON Text.vim"("Anything"=w282) -> ("<JSON>"=w278:string)  [unwired: 9 in, 1 out]
          n95 = case shown="\"Double\"" w281 {
            tunnel: w280 -> [w292 w303 w386 w470 w552 w636 w720]
            tunnel: w279 -> [w291 w302 w385 w468 w551 w634 w718]
            tunnel: w278 -> [w290 w301 w384 w467 w550 w633 w717]
            tunnel: w277 -> [w294 w300 w383 w466 w549 w632 w714]
            tunnel: w276 -> [_ w298 w387 w464 w547 w630 _]
            tunnel: [string[] ["name", "description-en", "documentation-en", "dataType", "bitfield", "access"] ("Item Names") w305 w388 w471 w554 w637 string[] ["name", "description-en", "documentation-en", "dataType", "bitfield", "access"] ("Item Names")] -> w274
            tunnel: [w286 w304 w381 w469 w553 w635 w719] -> w273
            tunnel: w275 -> [w285 w299 w382 w465 w548 w631 w713]
            tunnel: w270 -> [_ w297 w380 w463 w546 w629 _]
            tunnel: w269 -> [_ w296 w379 w462 w545 w628 _]
            frame "String", Default {
              n96 = call "To JSON Text.vim"("Anything"="String") -> ("<JSON>"=w289:string)  [unwired: 9 in, 1 out]
              n97 = call "To JSON Text.vim"("Anything"=w294) -> ("<JSON>"=w288:string)  [unwired: 9 in, 1 out]
              n98 = call "To JSON Text.vim"("Anything"=w285) -> ("<JSON>"=w287:string)  [unwired: 9 in, 1 out]
              n99 = Build Array(w292, w291, w290, w289, w288, w287) -> (w286:string[])
            }
            frame "Double" {
              n100 = case shown="True" w296 {
                tunnel: [w325 w361] -> w305
                tunnel: [w324 w360] -> w304
                tunnel: w303 -> [w323 w359]
                tunnel: w302 -> [w322 w358]
                tunnel: w301 -> [w321 w357]
                tunnel: w300 -> [w318 w354]
                tunnel: w299 -> [w317 w353]
                tunnel: w298 -> [w314 _]
                tunnel: w297 -> [w307 w348]
                frame True {
                  n101 = Unbundle By Name(w314) -> ("Min(Double)"=w313:dbl, "Max(Double)"=w312:dbl)
                  n102 = Equal?(x=w307, y="NoScale") -> (x = y?=w308:bool)
                  n103 = call "To JSON Text.vim"("Anything"="Double") -> ("<JSON>"=w319:string)  [unwired: 9 in, 1 out]
                  n104 = call "To JSON Text.vim"("Anything"=w318) -> ("<JSON>"=w316:string)  [unwired: 9 in, 1 out]
                  n105 = call "To JSON Text.vim"("Anything"=w317) -> ("<JSON>"=w315:string)  [unwired: 9 in, 1 out]
                  n106 = call "To JSON Text.vim"("Anything"=w313) -> ("<JSON>"=w311:string)  [unwired: 9 in, 1 out]
                  n107 = call "To JSON Text.vim"("Anything"=w312) -> ("<JSON>"=w310:string)  [unwired: 9 in, 1 out]
                  n108 = call "To JSON Text.vim"("Anything"=w307) -> ("<JSON>"=w306:string)  [unwired: 9 in, 1 out]
                  n109 = case shown="False" w308 {
                    tunnel: [string[] ["name", "description-en", "documentation-en", "dataType", "bitfield", "access", "min", "max", "scale"] ("Item Names") string[] ["name", "description-en", "documentation-en", "dataType", "bitfield", "access", "min", "max"] ("Item Names")] -> w325
                    tunnel: [w327 w345] -> w324
                    tunnel: w323 -> [w336 w344]
                    tunnel: w322 -> [w335 w343]
                    tunnel: w321 -> [w334 w342]
                    tunnel: w319 -> [w333 w341]
                    tunnel: w316 -> [w332 w340]
                    tunnel: w315 -> [w331 w339]
                    tunnel: w311 -> [w330 w338]
                    tunnel: w310 -> [w329 w337]
                    tunnel: w306 -> [w328 _]
                    frame False {
                      n110 = Build Array(w336, w335, w334, w333, w332, w331, w330, w329, w328) -> (w327:string[])
                    }
                    frame True {
                      n111 = Build Array(w344, w343, w342, w341, w340, w339, w338, w337) -> (w345:string[])
                    }
                  }
                }
                frame False {
                  n112 = Equal?(x=w348, y="NoScale") -> (x = y?=w349:bool)
                  n113 = call "To JSON Text.vim"("Anything"="Double") -> ("<JSON>"=w355:string)  [unwired: 9 in, 1 out]
                  n114 = call "To JSON Text.vim"("Anything"=w354) -> ("<JSON>"=w352:string)  [unwired: 9 in, 1 out]
                  n115 = call "To JSON Text.vim"("Anything"=w353) -> ("<JSON>"=w351:string)  [unwired: 9 in, 1 out]
                  n116 = call "To JSON Text.vim"("Anything"=w348) -> ("<JSON>"=w347:string)  [unwired: 9 in, 1 out]
                  n117 = case shown="False" w349 {
                    tunnel: [string[] ["name", "description-en", "documentation-en", "dataType", "bitfield", "access", "scale"] ("Item Names") string[] ["name", "description-en", "documentation-en", "dataType", "bitfield", "access"] ("Item Names")] -> w361
                    tunnel: [w364 w377] -> w360
                    tunnel: w359 -> [w370 w376]
                    tunnel: w358 -> [w369 w375]
                    tunnel: w357 -> [w368 w374]
                    tunnel: w355 -> [w367 w373]
                    tunnel: w352 -> [w366 w372]
                    tunnel: w351 -> [w365 w371]
                    tunnel: w347 -> [w362 _]
                    frame False {
                      n118 = Build Array(w370, w369, w368, w367, w366, w365, w362) -> (w364:string[])
                    }
                    frame True {
                      n119 = Build Array(w376, w375, w374, w373, w372, w371) -> (w377:string[])
                    }
                  }
                }
              }
            }
            frame "U64" {
              n120 = case shown="True" w379 {
                tunnel: [w408 w444] -> w388
                tunnel: w387 -> [w407 _]
                tunnel: w386 -> [w402 w443]
                tunnel: w385 -> [w401 w442]
                tunnel: w384 -> [w400 w441]
                tunnel: w383 -> [w398 w439]
                tunnel: w382 -> [w397 w438]
                tunnel: [w393 w434] -> w381
                tunnel: w380 -> [w391 w432]
                frame True {
                  n121 = Unbundle By Name(w407) -> ("Min(U64)"=w406:u64, "Max(U64)"=w405:u64)
                  n122 = Equal?(x=w391, y="NoScale") -> (x = y?=w390:bool)
                  n123 = call "To JSON Text.vim"("Anything"=w397) -> ("<JSON>"=w394:string)  [unwired: 9 in, 1 out]
                  n124 = call "To JSON Text.vim"("Anything"="UInt64") -> ("<JSON>"=w396:string)  [unwired: 9 in, 1 out]
                  n125 = call "To JSON Text.vim"("Anything"=w398) -> ("<JSON>"=w395:string)  [unwired: 9 in, 1 out]
                  n126 = call "To JSON Text.vim"("Anything"=w406) -> ("<JSON>"=w404:string)  [unwired: 9 in, 1 out]
                  n127 = call "To JSON Text.vim"("Anything"=w405) -> ("<JSON>"=w403:string)  [unwired: 9 in, 1 out]
                  n128 = call "To JSON Text.vim"("Anything"=w391) -> ("<JSON>"=w389:string)  [unwired: 9 in, 1 out]
                  n129 = case shown="True" w390 {
                    tunnel: [string[] ["name", "description-en", "documentation-en", "dataType", "bitfield", "access", "min", "max", "scale"] ("Item Names") string[] ["name", "description-en", "documentation-en", "dataType", "bitfield", "access", "min", "max"] ("Item Names")] -> w408
                    tunnel: w404 -> [w412 w428]
                    tunnel: w403 -> [w411 w427]
                    tunnel: w402 -> [w418 w426]
                    tunnel: w401 -> [w417 w425]
                    tunnel: w400 -> [w416 w424]
                    tunnel: w396 -> [w415 w423]
                    tunnel: w395 -> [w414 w422]
                    tunnel: w394 -> [w413 w421]
                    tunnel: [w409 w420] -> w393
                    tunnel: w389 -> [w410 _]
                    frame False {
                      n130 = Build Array(w418, w417, w416, w415, w414, w413, w412, w411, w410) -> (w409:string[])
                    }
                    frame True {
                      n131 = Build Array(w426, w425, w424, w423, w422, w421, w428, w427) -> (w420:string[])
                    }
                  }
                }
                frame False {
                  n132 = Equal?(x=w432, y="NoScale") -> (x = y?=w431:bool)
                  n133 = call "To JSON Text.vim"("Anything"=w438) -> ("<JSON>"=w435:string)  [unwired: 9 in, 1 out]
                  n134 = call "To JSON Text.vim"("Anything"="UInt64") -> ("<JSON>"=w437:string)  [unwired: 9 in, 1 out]
                  n135 = call "To JSON Text.vim"("Anything"=w439) -> ("<JSON>"=w436:string)  [unwired: 9 in, 1 out]
                  n136 = call "To JSON Text.vim"("Anything"=w432) -> ("<JSON>"=w430:string)  [unwired: 9 in, 1 out]
                  n137 = case shown="True" w431 {
                    tunnel: [string[] ["name", "description-en", "documentation-en", "dataType", "bitfield", "access", "scale"] ("Item Names") string[] ["name", "description-en", "documentation-en", "dataType", "bitfield", "access"] ("Item Names")] -> w444
                    tunnel: w443 -> [w452 w460]
                    tunnel: w442 -> [w451 w459]
                    tunnel: w441 -> [w450 w458]
                    tunnel: w437 -> [w449 w457]
                    tunnel: w436 -> [w448 w456]
                    tunnel: w435 -> [w447 w455]
                    tunnel: [w446 w454] -> w434
                    tunnel: w430 -> [w445 _]
                    frame False {
                      n138 = Build Array(w452, w451, w450, w449, w448, w447, w445) -> (w446:string[])
                    }
                    frame True {
                      n139 = Build Array(w460, w459, w458, w457, w456, w455) -> (w454:string[])
                    }
                  }
                }
              }
            }
            frame "I64" {
              n140 = case shown="True" w462 {
                tunnel: [w491 w527] -> w471
                tunnel: w470 -> [w490 w526]
                tunnel: [w489 w525] -> w469
                tunnel: w468 -> [w488 w524]
                tunnel: w467 -> [w487 w523]
                tunnel: w466 -> [w485 w521]
                tunnel: w465 -> [w484 w520]
                tunnel: w464 -> [w480 _]
                tunnel: w463 -> [w474 w515]
                frame True {
                  n141 = Unbundle By Name(w480) -> ("Min(I64)"=w479:i64, "Max(I64)"=w478:i64)
                  n142 = call "To JSON Text.vim"("Anything"="Int64") -> ("<JSON>"=w483:string)  [unwired: 9 in, 1 out]
                  n143 = call "To JSON Text.vim"("Anything"=w485) -> ("<JSON>"=w482:string)  [unwired: 9 in, 1 out]
                  n144 = call "To JSON Text.vim"("Anything"=w484) -> ("<JSON>"=w481:string)  [unwired: 9 in, 1 out]
                  n145 = Equal?(x=w474, y="NoScale") -> (x = y?=w473:bool)
                  n146 = call "To JSON Text.vim"("Anything"=w479) -> ("<JSON>"=w477:string)  [unwired: 9 in, 1 out]
                  n147 = call "To JSON Text.vim"("Anything"=w478) -> ("<JSON>"=w476:string)  [unwired: 9 in, 1 out]
                  n148 = call "To JSON Text.vim"("Anything"=w474) -> ("<JSON>"=w472:string)  [unwired: 9 in, 1 out]
                  n149 = case shown="True" w473 {
                    tunnel: [string[] ["name", "description-en", "documentation-en", "dataType", "bitfield", "access", "min", "max", "scale"] ("Item Names") string[] ["name", "description-en", "documentation-en", "dataType", "bitfield", "access", "min", "max"] ("Item Names")] -> w491
                    tunnel: w490 -> [w502 w511]
                    tunnel: [w493 w510] -> w489
                    tunnel: w488 -> [w501 w509]
                    tunnel: w487 -> [w500 w508]
                    tunnel: w483 -> [w499 w507]
                    tunnel: w482 -> [w498 w506]
                    tunnel: w481 -> [w497 w505]
                    tunnel: w477 -> [w496 w504]
                    tunnel: w476 -> [w495 w503]
                    tunnel: w472 -> [w492 _]
                    frame False {
                      n150 = Build Array(w502, w501, w500, w499, w498, w497, w496, w495, w492) -> (w493:string[])
                    }
                    frame True {
                      n151 = Build Array(w511, w509, w508, w507, w506, w505, w504, w503) -> (w510:string[])
                    }
                  }
                }
                frame False {
                  n152 = call "To JSON Text.vim"("Anything"="Int64") -> ("<JSON>"=w519:string)  [unwired: 9 in, 1 out]
                  n153 = call "To JSON Text.vim"("Anything"=w521) -> ("<JSON>"=w518:string)  [unwired: 9 in, 1 out]
                  n154 = call "To JSON Text.vim"("Anything"=w520) -> ("<JSON>"=w517:string)  [unwired: 9 in, 1 out]
                  n155 = Equal?(x=w515, y="NoScale") -> (x = y?=w514:bool)
                  n156 = call "To JSON Text.vim"("Anything"=w515) -> ("<JSON>"=w513:string)  [unwired: 9 in, 1 out]
                  n157 = case shown="True" w514 {
                    tunnel: [string[] ["name", "description-en", "documentation-en", "dataType", "bitfield", "access", "scale"] ("Item Names") string[] ["name", "description-en", "documentation-en", "dataType", "bitfield", "access"] ("Item Names")] -> w527
                    tunnel: w526 -> [w536 w543]
                    tunnel: [w529 w542] -> w525
                    tunnel: w524 -> [w535 w541]
                    tunnel: w523 -> [w534 w540]
                    tunnel: w519 -> [w533 w539]
                    tunnel: w518 -> [w532 w538]
                    tunnel: w517 -> [w531 w537]
                    tunnel: w513 -> [w528 _]
                    frame False {
                      n158 = Build Array(w536, w535, w534, w533, w532, w531, w528) -> (w529:string[])
                    }
                    frame True {
                      n159 = Build Array(w543, w541, w540, w539, w538, w537) -> (w542:string[])
                    }
                  }
                }
              }
            }
            frame "U32" {
              n160 = case shown="True" w545 {
                tunnel: [w574 w610] -> w554
                tunnel: [w573 w609] -> w553
                tunnel: w552 -> [w572 w608]
                tunnel: w551 -> [w571 w607]
                tunnel: w550 -> [w570 w606]
                tunnel: w549 -> [w563 w603]
                tunnel: w548 -> [w561 w601]
                tunnel: w547 -> [w559 _]
                tunnel: w546 -> [w557 w598]
                frame True {
                  n161 = Unbundle By Name(w559) -> ("Min(U32)"=w569:u32, "Max(U32)"=w568:u32)
                  n162 = call "To JSON Text.vim"("Anything"=w563) -> ("<JSON>"=w562:string)  [unwired: 9 in, 1 out]
                  n163 = call "To JSON Text.vim"("Anything"=w561) -> ("<JSON>"=w560:string)  [unwired: 9 in, 1 out]
                  n164 = call "To JSON Text.vim"("Anything"="UInt32") -> ("<JSON>"=w564:string)  [unwired: 9 in, 1 out]
                  n165 = Equal?(x=w557, y="NoScale") -> (x = y?=w555:bool)
                  n166 = call "To JSON Text.vim"("Anything"=w569) -> ("<JSON>"=w567:string)  [unwired: 9 in, 1 out]
                  n167 = call "To JSON Text.vim"("Anything"=w568) -> ("<JSON>"=w566:string)  [unwired: 9 in, 1 out]
                  n168 = call "To JSON Text.vim"("Anything"=w557) -> ("<JSON>"=w556:string)  [unwired: 9 in, 1 out]
                  n169 = case shown="True" w555 {
                    tunnel: [string[] ["name", "description-en", "documentation-en", "dataType", "bitfield", "access", "min", "max", "scale"] ("Item Names") string[] ["name", "description-en", "documentation-en", "dataType", "bitfield", "access", "min", "max"] ("Item Names")] -> w574
                    tunnel: [w584 w594] -> w573
                    tunnel: w572 -> [w583 w593]
                    tunnel: w571 -> [w582 w592]
                    tunnel: w570 -> [w581 w591]
                    tunnel: w567 -> [w577 w590]
                    tunnel: w566 -> [w576 w589]
                    tunnel: w564 -> [w580 w588]
                    tunnel: w562 -> [w579 w587]
                    tunnel: w560 -> [w578 w586]
                    tunnel: w556 -> [w575 _]
                    frame False {
                      n170 = Build Array(w583, w582, w581, w580, w579, w578, w577, w576, w575) -> (w584:string[])
                    }
                    frame True {
                      n171 = Build Array(w593, w592, w591, w588, w587, w586, w590, w589) -> (w594:string[])
                    }
                  }
                }
                frame False {
                  n172 = call "To JSON Text.vim"("Anything"=w603) -> ("<JSON>"=w602:string)  [unwired: 9 in, 1 out]
                  n173 = call "To JSON Text.vim"("Anything"=w601) -> ("<JSON>"=w600:string)  [unwired: 9 in, 1 out]
                  n174 = call "To JSON Text.vim"("Anything"="UInt32") -> ("<JSON>"=w604:string)  [unwired: 9 in, 1 out]
                  n175 = Equal?(x=w598, y="NoScale") -> (x = y?=w596:bool)
                  n176 = call "To JSON Text.vim"("Anything"=w598) -> ("<JSON>"=w597:string)  [unwired: 9 in, 1 out]
                  n177 = case shown="False" w596 {
                    tunnel: [string[] ["name", "description-en", "documentation-en", "dataType", "bitfield", "access", "scale"] ("Item Names") string[] ["name", "description-en", "documentation-en", "dataType", "bitfield", "access"] ("Item Names")] -> w610
                    tunnel: [w618 w626] -> w609
                    tunnel: w608 -> [w617 w625]
                    tunnel: w607 -> [w616 w624]
                    tunnel: w606 -> [w615 w623]
                    tunnel: w604 -> [w614 w622]
                    tunnel: w602 -> [w613 w621]
                    tunnel: w600 -> [w612 w620]
                    tunnel: w597 -> [w611 _]
                    frame False {
                      n178 = Build Array(w617, w616, w615, w614, w613, w612, w611) -> (w618:string[])
                    }
                    frame True {
                      n179 = Build Array(w625, w624, w623, w622, w621, w620) -> (w626:string[])
                    }
                  }
                }
              }
            }
            frame "I32" {
              n180 = case shown="True" w628 {
                tunnel: [w657 w693] -> w637
                tunnel: w636 -> [w656 w692]
                tunnel: [w655 w691] -> w635
                tunnel: w634 -> [w654 w690]
                tunnel: w633 -> [w653 w689]
                tunnel: w632 -> [w646 w686]
                tunnel: w631 -> [w645 w685]
                tunnel: w630 -> [w642 _]
                tunnel: w629 -> [w640 w681]
                frame True {
                  n181 = Unbundle By Name(w642) -> ("Min(I32)"=w652:i32, "Max(I32)"=w651:i32)
                  n182 = call "To JSON Text.vim"("Anything"=w645) -> ("<JSON>"=w643:string)  [unwired: 9 in, 1 out]
                  n183 = call "To JSON Text.vim"("Anything"="Int32") -> ("<JSON>"=w647:string)  [unwired: 9 in, 1 out]
                  n184 = call "To JSON Text.vim"("Anything"=w646) -> ("<JSON>"=w644:string)  [unwired: 9 in, 1 out]
                  n185 = Equal?(x=w640, y="NoScale") -> (x = y?=w639:bool)
                  n186 = call "To JSON Text.vim"("Anything"=w640) -> ("<JSON>"=w638:string)  [unwired: 9 in, 1 out]
                  n187 = call "To JSON Text.vim"("Anything"=w651) -> ("<JSON>"=w649:string)  [unwired: 9 in, 1 out]
                  n188 = call "To JSON Text.vim"("Anything"=w652) -> ("<JSON>"=w650:string)  [unwired: 9 in, 1 out]
                  n189 = case shown="True" w639 {
                    tunnel: [string[] ["name", "description-en", "documentation-en", "dataType", "bitfield", "access", "min", "max", "scale"] ("Item Names") string[] ["name", "description-en", "documentation-en", "dataType", "bitfield", "access", "min", "max"] ("Item Names")] -> w657
                    tunnel: w656 -> [w667 w677]
                    tunnel: [w658 w676] -> w655
                    tunnel: w654 -> [w666 w675]
                    tunnel: w653 -> [w665 w674]
                    tunnel: w650 -> [w661 w673]
                    tunnel: w649 -> [w660 w672]
                    tunnel: w647 -> [w664 w671]
                    tunnel: w644 -> [w663 w670]
                    tunnel: w643 -> [w662 w669]
                    tunnel: w638 -> [w659 _]
                    frame False {
                      n190 = Build Array(w667, w666, w665, w664, w663, w662, w661, w660, w659) -> (w658:string[])
                    }
                    frame True {
                      n191 = Build Array(w677, w675, w674, w671, w670, w669, w673, w672) -> (w676:string[])
                    }
                  }
                }
                frame False {
                  n192 = call "To JSON Text.vim"("Anything"=w685) -> ("<JSON>"=w683:string)  [unwired: 9 in, 1 out]
                  n193 = call "To JSON Text.vim"("Anything"="Int32") -> ("<JSON>"=w687:string)  [unwired: 9 in, 1 out]
                  n194 = call "To JSON Text.vim"("Anything"=w686) -> ("<JSON>"=w684:string)  [unwired: 9 in, 1 out]
                  n195 = Equal?(x=w681, y="NoScale") -> (x = y?=w680:bool)
                  n196 = call "To JSON Text.vim"("Anything"=w681) -> ("<JSON>"=w679:string)  [unwired: 9 in, 1 out]
                  n197 = case shown="True" w680 {
                    tunnel: [string[] ["name", "description-en", "documentation-en", "dataType", "bitfield", "access", "scale"] ("Item Names") string[] ["name", "description-en", "documentation-en", "dataType", "bitfield", "access"] ("Item Names")] -> w693
                    tunnel: w692 -> [w701 w709]
                    tunnel: [w695 w708] -> w691
                    tunnel: w690 -> [w700 w707]
                    tunnel: w689 -> [w699 w706]
                    tunnel: w687 -> [w698 w705]
                    tunnel: w684 -> [w697 w704]
                    tunnel: w683 -> [w696 w703]
                    tunnel: w679 -> [w694 _]
                    frame False {
                      n198 = Build Array(w701, w700, w699, w698, w697, w696, w694) -> (w695:string[])
                    }
                    frame True {
                      n199 = Build Array(w709, w707, w706, w705, w704, w703) -> (w708:string[])
                    }
                  }
                }
              }
            }
            frame "Bool" {
              n200 = call "To JSON Text.vim"("Anything"=w714) -> ("<JSON>"=w712:string)  [unwired: 9 in, 1 out]
              n201 = call "To JSON Text.vim"("Anything"="Bool") -> ("<JSON>"=w715:string)  [unwired: 9 in, 1 out]
              n202 = call "To JSON Text.vim"("Anything"=w713) -> ("<JSON>"=w711:string)  [unwired: 9 in, 1 out]
              n203 = Build Array(w720, w718, w717, w715, w712, w711) -> (w719:string[])
            }
          }
        }
      }
      n204 = Unbundle By Name(w34) -> ("Property Index"=w33:i32)
      n205 = Unbundle By Name(w27) -> ("Ref Cluster.Property tree"=w29:refnum<vi>)
      n206 = Unbundle By Name(w30) -> ("NewPropertyParameter.Name"=w26:string)
      n207 = Build Array(w26) -> (w28:string[])
      n208 = property class="Tree (strict)"(reference=w29, "Value"=w28) -> ()  [unwired: 1 in, 2 out]
      n209 = Bundle By Name(cluster=w27, "Selected Type and name.Selected Property Name"=w26) -> (w25:T2)
      n210 = call "InsertIntoNewProperty.vi"("$Path or Item Name"="$.properties" ("string"), "JSON Items"=w21, "JSON In"=w23, "error in (no error)"=w17, "Item Names"=w22, "index"=w33, "Input array"=w20) -> ("error out"=w18:errorcluster, "<JSON>"=w19:string)  [unwired: 3 in]
    }
    frame "Physical Channel" {
      n211 = case shown="False" w754 {
        tunnel: w753 -> [_ w989]
        tunnel: w752 -> [w755 w988]
        tunnel: [w764 w987] -> w734
        tunnel: [w763 w986] -> w733
        tunnel: w743 -> [w762 w985]
        tunnel: w745 -> [_ w984]
        tunnel: w744 -> [w756 w983]
        frame False {
          n212 = Unbundle By Name(w762) -> ("NewPropertyParameter.Name"=w761:string, "NewPropertyParameter.Description"=w760:string, "NewPropertyParameter.Documentation"=w759:string, "NewPropertyParameter.DataType"=w765:T13, "NewPropertyParameter.Value_Cluster"=w766:T14, "Min_Max_Cluster"=w767:T15)
          n213 = call "To JSON Text.vim"("Anything"=w761) -> ("<JSON>"=w768:string)  [unwired: 9 in, 1 out]
          n214 = call "To JSON Text.vim"("Anything"=w760) -> ("<JSON>"=w758:string)  [unwired: 9 in, 1 out]
          n215 = call "To JSON Text.vim"("Anything"=w759) -> ("<JSON>"=w757:string)  [unwired: 9 in, 1 out]
          n216 = case shown="\"I64\"" w765 {
            tunnel: w766 -> [w780 w789 w827 w864 w901 w939 w980]
            tunnel: w768 -> [w773 w785 w823 w860 w898 w936 w974]
            tunnel: [string[] ["name", "description-en", "documentation-en", "dataType", "value", "access"] ("Item Names") w787 w825 w862 w902 w940 string[] ["name", "description-en", "documentation-en", "dataType", "value", "access"] ("Item Names")] -> w764
            tunnel: [w774 w788 w826 w863 w899 w937 w976] -> w763
            tunnel: w767 -> [_ w786 w824 w861 w900 w938 _]
            tunnel: w758 -> [w772 w784 w822 w859 w897 w935 w973]
            tunnel: w757 -> [w771 w783 w821 w858 w896 w934 w972]
            tunnel: w756 -> [_ w782 w820 w857 w895 w933 _]
            tunnel: w755 -> [w770 w781 w819 w856 w894 w932 w971]
            frame "String", Default {
              n217 = Unbundle By Name(w780) -> ("String"=w779:string)
              n218 = call "To JSON Text.vim"("Anything"="String") -> ("<JSON>"=w776:string)  [unwired: 9 in, 1 out]
              n219 = call "To JSON Text.vim"("Anything"=w779) -> ("<JSON>"=w775:string)  [unwired: 9 in, 1 out]
              n220 = call "To JSON Text.vim"("Anything"=w770) -> ("<JSON>"=w769:string)  [unwired: 9 in, 1 out]
              n221 = Build Array(w773, w772, w771, w776, w775, w769) -> (w774:string[])
            }
            frame "Double" {
              n222 = case shown="True" w782 {
                tunnel: w789 -> [w806 w818]
                tunnel: [w801 w813] -> w788
                tunnel: [string[] ["name", "description-en", "documentation-en", "dataType", "value", "min", "max", "access"] ("Item Names") string[] ["name", "description-en", "documentation-en", "dataType", "value", "access"] ("Item Names")] -> w787
                tunnel: w786 -> [w799 _]
                tunnel: w785 -> [w794 w811]
                tunnel: w784 -> [w793 w810]
                tunnel: w783 -> [w792 w809]
                tunnel: w781 -> [w791 w808]
                frame True {
                  n223 = Unbundle By Name(w799) -> ("Min(Double)"=w798:dbl, "Max(Double)"=w797:dbl)
                  n224 = Unbundle By Name(w806) -> ("DBL"=w805:dbl)
                  n225 = call "To JSON Text.vim"("Anything"="Double") -> ("<JSON>"=w803:string)  [unwired: 9 in, 1 out]
                  n226 = call "To JSON Text.vim"("Anything"=w805) -> ("<JSON>"=w802:string)  [unwired: 9 in, 1 out]
                  n227 = call "To JSON Text.vim"("Anything"=w798) -> ("<JSON>"=w796:string)  [unwired: 9 in, 1 out]
                  n228 = call "To JSON Text.vim"("Anything"=w797) -> ("<JSON>"=w795:string)  [unwired: 9 in, 1 out]
                  n229 = call "To JSON Text.vim"("Anything"=w791) -> ("<JSON>"=w790:string)  [unwired: 9 in, 1 out]
                  n230 = Build Array(w794, w793, w792, w803, w802, w796, w795, w790) -> (w801:string[])
                }
                frame False {
                  n231 = Unbundle By Name(w818) -> ("DBL"=w817:dbl)
                  n232 = call "To JSON Text.vim"("Anything"=w808) -> ("<JSON>"=w807:string)  [unwired: 9 in, 1 out]
                  n233 = call "To JSON Text.vim"("Anything"="Double") -> ("<JSON>"=w815:string)  [unwired: 9 in, 1 out]
                  n234 = call "To JSON Text.vim"("Anything"=w817) -> ("<JSON>"=w814:string)  [unwired: 9 in, 1 out]
                  n235 = Build Array(w811, w810, w809, w815, w814, w807) -> (w813:string[])
                }
              }
            }
            frame "U64" {
              n236 = case shown="True" w820 {
                tunnel: w827 -> [w844 w855]
                tunnel: [w839 w850] -> w826
                tunnel: [string[] ["name", "description-en", "documentation-en", "dataType", "value", "min", "max", "access"] ("Item Names") string[] ["name", "description-en", "documentation-en", "dataType", "value", "access"] ("Item Names")] -> w825
                tunnel: w824 -> [w837 _]
                tunnel: w823 -> [w832 w848]
                tunnel: w822 -> [w831 w847]
                tunnel: w821 -> [w830 w846]
                tunnel: w819 -> [w829 w845]
                frame True {
                  n237 = Unbundle By Name(w844) -> ("U64"=w843:u64)
                  n238 = Unbundle By Name(w837) -> ("Min(U64)"=w836:u64, "Max(U64)"=w835:u64)
                  n239 = call "To JSON Text.vim"("Anything"="UInt64") -> ("<JSON>"=w841:string)  [unwired: 9 in, 1 out]
                  n240 = call "To JSON Text.vim"("Anything"=w843) -> ("<JSON>"=w840:string)  [unwired: 9 in, 1 out]
                  n241 = call "To JSON Text.vim"("Anything"=w836) -> ("<JSON>"=w834:string)  [unwired: 9 in, 1 out]
                  n242 = call "To JSON Text.vim"("Anything"=w835) -> ("<JSON>"=w833:string)  [unwired: 9 in, 1 out]
                  n243 = call "To JSON Text.vim"("Anything"=w829) -> ("<JSON>"=w828:string)  [unwired: 9 in, 1 out]
                  n244 = Build Array(w832, w831, w830, w841, w840, w834, w833, w828) -> (w839:string[])
                }
                frame False {
                  n245 = Unbundle By Name(w855) -> ("U64"=w854:u64)
                  n246 = call "To JSON Text.vim"("Anything"="UInt64") -> ("<JSON>"=w852:string)  [unwired: 9 in, 1 out]
                  n247 = call "To JSON Text.vim"("Anything"=w854) -> ("<JSON>"=w851:string)  [unwired: 9 in, 1 out]
                  n248 = Build Array(w848, w847, w846, w852, w851, w845) -> (w850:string[])
                }
              }
            }
            frame "I64" {
              n249 = case shown="False" w857 {
                tunnel: w864 -> [w881 w893]
                tunnel: [w876 w888] -> w863
                tunnel: [string[] ["name", "description-en", "documentation-en", "dataType", "value", "min", "max", "access"] ("Item Names") string[] ["name", "description-en", "documentation-en", "dataType", "value", "access"] ("Item Names")] -> w862
                tunnel: w861 -> [w874 _]
                tunnel: w860 -> [w869 w886]
                tunnel: w859 -> [w868 w885]
                tunnel: w858 -> [w867 w884]
                tunnel: w856 -> [w866 w883]
                frame True {
                  n250 = Unbundle By Name(w881) -> ("I64"=w880:i64)
                  n251 = Unbundle By Name(w874) -> ("Min(I64)"=w873:i64, "Max(I64)"=w872:i64)
                  n252 = call "To JSON Text.vim"("Anything"=w866) -> ("<JSON>"=w865:string)  [unwired: 9 in, 1 out]
                  n253 = call "To JSON Text.vim"("Anything"="Int64") -> ("<JSON>"=w878:string)  [unwired: 9 in, 1 out]
                  n254 = call "To JSON Text.vim"("Anything"=w880) -> ("<JSON>"=w877:string)  [unwired: 9 in, 1 out]
                  n255 = call "To JSON Text.vim"("Anything"=w873) -> ("<JSON>"=w871:string)  [unwired: 9 in, 1 out]
                  n256 = call "To JSON Text.vim"("Anything"=w872) -> ("<JSON>"=w870:string)  [unwired: 9 in, 1 out]
                  n257 = Build Array(w869, w868, w867, w878, w877, w871, w870, w865) -> (w876:string[])
                }
                frame False {
                  n258 = Unbundle By Name(w893) -> ("I64"=w892:i64)
                  n259 = call "To JSON Text.vim"("Anything"="Int64") -> ("<JSON>"=w890:string)  [unwired: 9 in, 1 out]
                  n260 = call "To JSON Text.vim"("Anything"=w892) -> ("<JSON>"=w889:string)  [unwired: 9 in, 1 out]
                  n261 = call "To JSON Text.vim"("Anything"=w883) -> ("<JSON>"=w882:string)  [unwired: 9 in, 1 out]
                  n262 = Build Array(w886, w885, w884, w890, w889, w882) -> (w888:string[])
                }
              }
            }
            frame "U32" {
              n263 = case shown="True" w895 {
                tunnel: [string[] ["name", "description-en", "documentation-en", "dataType", "value", "min", "max", "access"] ("Item Names") string[] ["name", "description-en", "documentation-en", "dataType", "value", "access"] ("Item Names")] -> w902
                tunnel: w901 -> [w916 w928]
                tunnel: w900 -> [w915 _]
                tunnel: [w908 w925] -> w899
                tunnel: w898 -> [w907 w924]
                tunnel: w897 -> [w906 w923]
                tunnel: w896 -> [w905 w922]
                tunnel: w894 -> [w904 w921]
                frame True {
                  n264 = Unbundle By Name(w915) -> ("Min(U32)"=w914:u32, "Max(U32)"=w913:u32)
                  n265 = Unbundle By Name(w916) -> ("U32"=w917:u32)
                  n266 = call "To JSON Text.vim"("Anything"="UInt32") -> ("<JSON>"=w912:string)  [unwired: 9 in, 1 out]
                  n267 = call "To JSON Text.vim"("Anything"=w917) -> ("<JSON>"=w911:string)  [unwired: 9 in, 1 out]
                  n268 = call "To JSON Text.vim"("Anything"=w914) -> ("<JSON>"=w910:string)  [unwired: 9 in, 1 out]
                  n269 = call "To JSON Text.vim"("Anything"=w913) -> ("<JSON>"=w909:string)  [unwired: 9 in, 1 out]
                  n270 = call "To JSON Text.vim"("Anything"=w904) -> ("<JSON>"=w903:string)  [unwired: 9 in, 1 out]
                  n271 = Build Array(w907, w906, w905, w912, w911, w910, w909, w903) -> (w908:string[])
                }
                frame False {
                  n272 = Unbundle By Name(w928) -> ("U32"=w929:u32)
                  n273 = call "To JSON Text.vim"("Anything"="UInt32") -> ("<JSON>"=w927:string)  [unwired: 9 in, 1 out]
                  n274 = call "To JSON Text.vim"("Anything"=w929) -> ("<JSON>"=w926:string)  [unwired: 9 in, 1 out]
                  n275 = call "To JSON Text.vim"("Anything"=w921) -> ("<JSON>"=w920:string)  [unwired: 9 in, 1 out]
                  n276 = Build Array(w924, w923, w922, w927, w926, w920) -> (w925:string[])
                }
              }
            }
            frame "I32" {
              n277 = case shown="True" w933 {
                tunnel: [string[] ["name", "description-en", "documentation-en", "dataType", "value", "min", "max", "access"] ("Item Names") string[] ["name", "description-en", "documentation-en", "dataType", "value", "access"] ("Item Names")] -> w940
                tunnel: w939 -> [w955 w967]
                tunnel: w938 -> [w953 _]
                tunnel: [w946 w963] -> w937
                tunnel: w936 -> [w945 w962]
                tunnel: w935 -> [w944 w961]
                tunnel: w934 -> [w943 w960]
                tunnel: w932 -> [w942 w959]
                frame True {
                  n278 = Unbundle By Name(w953) -> ("Min(I32)"=w950:i32, "Max(I32)"=w949:i32)
                  n279 = Unbundle By Name(w955) -> ("I32"=w954:i32)
                  n280 = call "To JSON Text.vim"("Anything"="Int32") -> ("<JSON>"=w952:string)  [unwired: 9 in, 1 out]
                  n281 = call "To JSON Text.vim"("Anything"=w954) -> ("<JSON>"=w951:string)  [unwired: 9 in, 1 out]
                  n282 = call "To JSON Text.vim"("Anything"=w950) -> ("<JSON>"=w948:string)  [unwired: 9 in, 1 out]
                  n283 = call "To JSON Text.vim"("Anything"=w949) -> ("<JSON>"=w947:string)  [unwired: 9 in, 1 out]
                  n284 = call "To JSON Text.vim"("Anything"=w942) -> ("<JSON>"=w941:string)  [unwired: 9 in, 1 out]
                  n285 = Build Array(w945, w944, w943, w952, w951, w948, w947, w941) -> (w946:string[])
                }
                frame False {
                  n286 = Unbundle By Name(w967) -> ("I32"=w966:i32)
                  n287 = call "To JSON Text.vim"("Anything"=w966) -> ("<JSON>"=w964:string)  [unwired: 9 in, 1 out]
                  n288 = call "To JSON Text.vim"("Anything"="Int32") -> ("<JSON>"=w965:string)  [unwired: 9 in, 1 out]
                  n289 = call "To JSON Text.vim"("Anything"=w959) -> ("<JSON>"=w958:string)  [unwired: 9 in, 1 out]
                  n290 = Build Array(w962, w961, w960, w965, w964, w958) -> (w963:string[])
                }
              }
            }
            frame "Bool" {
              n291 = Unbundle By Name(w980) -> ("Ring"=w979:u16)
              n292 = Greater Than 0?(x=w979) -> (x > 0?=w975:bool)
              n293 = call "To JSON Text.vim"("Anything"="Bool") -> ("<JSON>"=w978:string)  [unwired: 9 in, 1 out]
              n294 = call "To JSON Text.vim"("Anything"=w975) -> ("<JSON>"=w977:string)  [unwired: 9 in, 1 out]
              n295 = call "To JSON Text.vim"("Anything"=w971) -> ("<JSON>"=w970:string)  [unwired: 9 in, 1 out]
              n296 = Build Array(w974, w973, w972, w978, w977, w970) -> (w976:string[])
            }
          }
        }
        frame True {
          n297 = Unbundle By Name(w985) -> ("NewPropertyParameter.Name"=w997:string, "NewPropertyParameter.Description"=w995:string, "NewPropertyParameter.Documentation"=w996:string, "NewPropertyParameter.DataType"=w991:T13, "Min_Max_Cluster"=w990:T15)
          n298 = call "To JSON Text.vim"("Anything"=w997) -> ("<JSON>"=w994:string)  [unwired: 9 in, 1 out]
          n299 = call "To JSON Text.vim"("Anything"=w995) -> ("<JSON>"=w993:string)  [unwired: 9 in, 1 out]
          n300 = call "To JSON Text.vim"("Anything"=w996) -> ("<JSON>"=w992:string)  [unwired: 9 in, 1 out]
          n301 = case shown="\"Double\", Default" w991 {
            tunnel: w994 -> [w1005 w1088 w1172 w1254 w1338 w1422]
            tunnel: w993 -> [w1004 w1087 w1170 w1253 w1336 w1420]
            tunnel: w992 -> [w1003 w1086 w1169 w1252 w1335 w1419]
            tunnel: w989 -> [w1002 w1085 w1168 w1251 w1334 w1416]
            tunnel: w990 -> [w1000 w1089 w1166 w1249 w1332 _]
            tunnel: [w1007 w1090 w1173 w1256 w1339 string[] ["name", "description-en", "documentation-en", "dataType", "bitfield", "access"] ("Item Names")] -> w987
            tunnel: [w1006 w1083 w1171 w1255 w1337 w1421] -> w986
            tunnel: w988 -> [w1001 w1084 w1167 w1250 w1333 w1415]
            tunnel: w984 -> [w999 w1082 w1165 w1248 w1331 _]
            tunnel: w983 -> [w998 w1081 w1164 w1247 w1330 _]
            frame "Double", Default {
              n302 = case shown="True" w998 {
                tunnel: [w1027 w1063] -> w1007
                tunnel: [w1026 w1062] -> w1006
                tunnel: w1005 -> [w1025 w1061]
                tunnel: w1004 -> [w1024 w1060]
                tunnel: w1003 -> [w1023 w1059]
                tunnel: w1002 -> [w1020 w1056]
                tunnel: w1001 -> [w1019 w1055]
                tunnel: w1000 -> [w1016 _]
                tunnel: w999 -> [w1010 w1051]
                frame True {
                  n303 = Unbundle By Name(w1016) -> ("Min(Double)"=w1015:dbl, "Max(Double)"=w1014:dbl)
                  n304 = call "To JSON Text.vim"("Anything"="Double") -> ("<JSON>"=w1021:string)  [unwired: 9 in, 1 out]
                  n305 = call "To JSON Text.vim"("Anything"=w1020) -> ("<JSON>"=w1018:string)  [unwired: 9 in, 1 out]
                  n306 = call "To JSON Text.vim"("Anything"=w1019) -> ("<JSON>"=w1017:string)  [unwired: 9 in, 1 out]
                  n307 = Equal?(x=w1010, y="NoScale") -> (x = y?=w1009:bool)
                  n308 = call "To JSON Text.vim"("Anything"=w1015) -> ("<JSON>"=w1013:string)  [unwired: 9 in, 1 out]
                  n309 = call "To JSON Text.vim"("Anything"=w1014) -> ("<JSON>"=w1012:string)  [unwired: 9 in, 1 out]
                  n310 = call "To JSON Text.vim"("Anything"=w1010) -> ("<JSON>"=w1008:string)  [unwired: 9 in, 1 out]
                  n311 = case shown="False" w1009 {
                    tunnel: [string[] ["name", "description-en", "documentation-en", "dataType", "bitfield", "access", "min", "max", "scale"] ("Item Names") string[] ["name", "description-en", "documentation-en", "dataType", "bitfield", "access", "min", "max"] ("Item Names")] -> w1027
                    tunnel: [w1037 w1047] -> w1026
                    tunnel: w1025 -> [w1036 w1046]
                    tunnel: w1024 -> [w1035 w1045]
                    tunnel: w1023 -> [w1034 w1044]
                    tunnel: w1021 -> [w1033 w1043]
                    tunnel: w1018 -> [w1032 w1042]
                    tunnel: w1017 -> [w1031 w1041]
                    tunnel: w1013 -> [w1030 w1040]
                    tunnel: w1012 -> [w1029 w1039]
                    tunnel: w1008 -> [w1028 _]
                    frame False {
                      n312 = Build Array(w1036, w1035, w1034, w1033, w1032, w1031, w1030, w1029, w1028) -> (w1037:string[])
                    }
                    frame True {
                      n313 = Build Array(w1046, w1045, w1044, w1043, w1042, w1041, w1040, w1039) -> (w1047:string[])
                    }
                  }
                }
                frame False {
                  n314 = call "To JSON Text.vim"("Anything"="Double") -> ("<JSON>"=w1057:string)  [unwired: 9 in, 1 out]
                  n315 = call "To JSON Text.vim"("Anything"=w1056) -> ("<JSON>"=w1054:string)  [unwired: 9 in, 1 out]
                  n316 = call "To JSON Text.vim"("Anything"=w1055) -> ("<JSON>"=w1053:string)  [unwired: 9 in, 1 out]
                  n317 = Equal?(x=w1051, y="NoScale") -> (x = y?=w1050:bool)
                  n318 = call "To JSON Text.vim"("Anything"=w1051) -> ("<JSON>"=w1049:string)  [unwired: 9 in, 1 out]
                  n319 = case shown="False" w1050 {
                    tunnel: [string[] ["name", "description-en", "documentation-en", "dataType", "bitfield", "access", "scale"] ("Item Names") string[] ["name", "description-en", "documentation-en", "dataType", "bitfield", "access"] ("Item Names")] -> w1063
                    tunnel: [w1071 w1079] -> w1062
                    tunnel: w1061 -> [w1070 w1078]
                    tunnel: w1060 -> [w1069 w1077]
                    tunnel: w1059 -> [w1068 w1076]
                    tunnel: w1057 -> [w1067 w1075]
                    tunnel: w1054 -> [w1066 w1074]
                    tunnel: w1053 -> [w1065 w1073]
                    tunnel: w1049 -> [w1064 _]
                    frame False {
                      n320 = Build Array(w1070, w1069, w1068, w1067, w1066, w1065, w1064) -> (w1071:string[])
                    }
                    frame True {
                      n321 = Build Array(w1078, w1077, w1076, w1075, w1074, w1073) -> (w1079:string[])
                    }
                  }
                }
              }
            }
            frame "U64" {
              n322 = case shown="True" w1081 {
                tunnel: [w1110 w1146] -> w1090
                tunnel: w1089 -> [w1109 _]
                tunnel: w1088 -> [w1104 w1145]
                tunnel: w1087 -> [w1103 w1144]
                tunnel: w1086 -> [w1102 w1143]
                tunnel: w1085 -> [w1100 w1141]
                tunnel: w1084 -> [w1099 w1140]
                tunnel: [w1095 w1136] -> w1083
                tunnel: w1082 -> [w1093 w1134]
                frame True {
                  n323 = Unbundle By Name(w1109) -> ("Min(U64)"=w1108:u64, "Max(U64)"=w1107:u64)
                  n324 = call "To JSON Text.vim"("Anything"=w1099) -> ("<JSON>"=w1096:string)  [unwired: 9 in, 1 out]
                  n325 = call "To JSON Text.vim"("Anything"="UInt64") -> ("<JSON>"=w1098:string)  [unwired: 9 in, 1 out]
                  n326 = call "To JSON Text.vim"("Anything"=w1100) -> ("<JSON>"=w1097:string)  [unwired: 9 in, 1 out]
                  n327 = Equal?(x=w1093, y="NoScale") -> (x = y?=w1092:bool)
                  n328 = call "To JSON Text.vim"("Anything"=w1108) -> ("<JSON>"=w1106:string)  [unwired: 9 in, 1 out]
                  n329 = call "To JSON Text.vim"("Anything"=w1107) -> ("<JSON>"=w1105:string)  [unwired: 9 in, 1 out]
                  n330 = call "To JSON Text.vim"("Anything"=w1093) -> ("<JSON>"=w1091:string)  [unwired: 9 in, 1 out]
                  n331 = case shown="False" w1092 {
                    tunnel: [string[] ["name", "description-en", "documentation-en", "dataType", "bitfield", "access", "min", "max", "scale"] ("Item Names") string[] ["name", "description-en", "documentation-en", "dataType", "bitfield", "access", "min", "max"] ("Item Names")] -> w1110
                    tunnel: w1106 -> [w1113 w1130]
                    tunnel: w1105 -> [w1112 w1129]
                    tunnel: w1104 -> [w1119 w1128]
                    tunnel: w1103 -> [w1118 w1127]
                    tunnel: w1102 -> [w1117 w1126]
                    tunnel: w1098 -> [w1116 w1125]
                    tunnel: w1097 -> [w1115 w1124]
                    tunnel: w1096 -> [w1114 w1123]
                    tunnel: [w1120 w1122] -> w1095
                    tunnel: w1091 -> [w1111 _]
                    frame False {
                      n332 = Build Array(w1119, w1118, w1117, w1116, w1115, w1114, w1113, w1112, w1111) -> (w1120:string[])
                    }
                    frame True {
                      n333 = Build Array(w1128, w1127, w1126, w1125, w1124, w1123, w1130, w1129) -> (w1122:string[])
                    }
                  }
                }
                frame False {
                  n334 = call "To JSON Text.vim"("Anything"=w1140) -> ("<JSON>"=w1137:string)  [unwired: 9 in, 1 out]
                  n335 = call "To JSON Text.vim"("Anything"="UInt64") -> ("<JSON>"=w1139:string)  [unwired: 9 in, 1 out]
                  n336 = call "To JSON Text.vim"("Anything"=w1141) -> ("<JSON>"=w1138:string)  [unwired: 9 in, 1 out]
                  n337 = Equal?(x=w1134, y="NoScale") -> (x = y?=w1133:bool)
                  n338 = call "To JSON Text.vim"("Anything"=w1134) -> ("<JSON>"=w1132:string)  [unwired: 9 in, 1 out]
                  n339 = case shown="False" w1133 {
                    tunnel: [string[] ["name", "description-en", "documentation-en", "dataType", "bitfield", "access", "scale"] ("Item Names") string[] ["name", "description-en", "documentation-en", "dataType", "bitfield", "access"] ("Item Names")] -> w1146
                    tunnel: w1145 -> [w1153 w1162]
                    tunnel: w1144 -> [w1152 w1161]
                    tunnel: w1143 -> [w1151 w1160]
                    tunnel: w1139 -> [w1150 w1159]
                    tunnel: w1138 -> [w1149 w1158]
                    tunnel: w1137 -> [w1148 w1157]
                    tunnel: [w1154 w1156] -> w1136
                    tunnel: w1132 -> [w1147 _]
                    frame False {
                      n340 = Build Array(w1153, w1152, w1151, w1150, w1149, w1148, w1147) -> (w1154:string[])
                    }
                    frame True {
                      n341 = Build Array(w1162, w1161, w1160, w1159, w1158, w1157) -> (w1156:string[])
                    }
                  }
                }
              }
            }
            frame "I64" {
              n342 = case shown="True" w1164 {
                tunnel: [w1193 w1229] -> w1173
                tunnel: w1172 -> [w1192 w1228]
                tunnel: [w1191 w1227] -> w1171
                tunnel: w1170 -> [w1190 w1226]
                tunnel: w1169 -> [w1189 w1225]
                tunnel: w1168 -> [w1187 w1223]
                tunnel: w1167 -> [w1186 w1222]
                tunnel: w1166 -> [w1182 _]
                tunnel: w1165 -> [w1176 w1217]
                frame True {
                  n343 = Unbundle By Name(w1182) -> ("Min(I64)"=w1181:i64, "Max(I64)"=w1180:i64)
                  n344 = call "To JSON Text.vim"("Anything"="Int64") -> ("<JSON>"=w1185:string)  [unwired: 9 in, 1 out]
                  n345 = call "To JSON Text.vim"("Anything"=w1187) -> ("<JSON>"=w1184:string)  [unwired: 9 in, 1 out]
                  n346 = call "To JSON Text.vim"("Anything"=w1186) -> ("<JSON>"=w1183:string)  [unwired: 9 in, 1 out]
                  n347 = Equal?(x=w1176, y="NoScale") -> (x = y?=w1175:bool)
                  n348 = call "To JSON Text.vim"("Anything"=w1180) -> ("<JSON>"=w1178:string)  [unwired: 9 in, 1 out]
                  n349 = call "To JSON Text.vim"("Anything"=w1181) -> ("<JSON>"=w1179:string)  [unwired: 9 in, 1 out]
                  n350 = call "To JSON Text.vim"("Anything"=w1176) -> ("<JSON>"=w1174:string)  [unwired: 9 in, 1 out]
                  n351 = case shown="False" w1175 {
                    tunnel: [string[] ["name", "description-en", "documentation-en", "dataType", "bitfield", "access", "min", "max", "scale"] ("Item Names") string[] ["name", "description-en", "documentation-en", "dataType", "bitfield", "access", "min", "max"] ("Item Names")] -> w1193
                    tunnel: w1192 -> [w1202 w1213]
                    tunnel: [w1203 w1212] -> w1191
                    tunnel: w1190 -> [w1201 w1211]
                    tunnel: w1189 -> [w1200 w1210]
                    tunnel: w1185 -> [w1199 w1209]
                    tunnel: w1184 -> [w1198 w1208]
                    tunnel: w1183 -> [w1197 w1207]
                    tunnel: w1179 -> [w1196 w1206]
                    tunnel: w1178 -> [w1195 w1205]
                    tunnel: w1174 -> [w1194 _]
                    frame False {
                      n352 = Build Array(w1202, w1201, w1200, w1199, w1198, w1197, w1196, w1195, w1194) -> (w1203:string[])
                    }
                    frame True {
                      n353 = Build Array(w1213, w1211, w1210, w1209, w1208, w1207, w1206, w1205) -> (w1212:string[])
                    }
                  }
                }
                frame False {
                  n354 = call "To JSON Text.vim"("Anything"="Int64") -> ("<JSON>"=w1221:string)  [unwired: 9 in, 1 out]
                  n355 = call "To JSON Text.vim"("Anything"=w1223) -> ("<JSON>"=w1220:string)  [unwired: 9 in, 1 out]
                  n356 = call "To JSON Text.vim"("Anything"=w1222) -> ("<JSON>"=w1219:string)  [unwired: 9 in, 1 out]
                  n357 = Equal?(x=w1217, y="NoScale") -> (x = y?=w1216:bool)
                  n358 = call "To JSON Text.vim"("Anything"=w1217) -> ("<JSON>"=w1215:string)  [unwired: 9 in, 1 out]
                  n359 = case shown="False" w1216 {
                    tunnel: [string[] ["name", "description-en", "documentation-en", "dataType", "bitfield", "access", "scale"] ("Item Names") string[] ["name", "description-en", "documentation-en", "dataType", "bitfield", "access"] ("Item Names")] -> w1229
                    tunnel: w1228 -> [w1236 w1245]
                    tunnel: [w1237 w1244] -> w1227
                    tunnel: w1226 -> [w1235 w1243]
                    tunnel: w1225 -> [w1234 w1242]
                    tunnel: w1221 -> [w1233 w1241]
                    tunnel: w1220 -> [w1232 w1240]
                    tunnel: w1219 -> [w1231 w1239]
                    tunnel: w1215 -> [w1230 _]
                    frame False {
                      n360 = Build Array(w1236, w1235, w1234, w1233, w1232, w1231, w1230) -> (w1237:string[])
                    }
                    frame True {
                      n361 = Build Array(w1245, w1243, w1242, w1241, w1240, w1239) -> (w1244:string[])
                    }
                  }
                }
              }
            }
            frame "U32" {
              n362 = case shown="False" w1247 {
                tunnel: [w1276 w1312] -> w1256
                tunnel: [w1275 w1311] -> w1255
                tunnel: w1254 -> [w1274 w1310]
                tunnel: w1253 -> [w1273 w1309]
                tunnel: w1252 -> [w1272 w1308]
                tunnel: w1251 -> [w1265 w1305]
                tunnel: w1250 -> [w1263 w1303]
                tunnel: w1249 -> [w1261 _]
                tunnel: w1248 -> [w1259 w1300]
                frame True {
                  n363 = Unbundle By Name(w1261) -> ("Min(U32)"=w1271:u32, "Max(U32)"=w1270:u32)
                  n364 = Equal?(x=w1259, y="NoScale") -> (x = y?=w1258:bool)
                  n365 = call "To JSON Text.vim"("Anything"=w1265) -> ("<JSON>"=w1264:string)  [unwired: 9 in, 1 out]
                  n366 = call "To JSON Text.vim"("Anything"=w1263) -> ("<JSON>"=w1262:string)  [unwired: 9 in, 1 out]
                  n367 = call "To JSON Text.vim"("Anything"="UInt32") -> ("<JSON>"=w1266:string)  [unwired: 9 in, 1 out]
                  n368 = call "To JSON Text.vim"("Anything"=w1259) -> ("<JSON>"=w1257:string)  [unwired: 9 in, 1 out]
                  n369 = call "To JSON Text.vim"("Anything"=w1271) -> ("<JSON>"=w1269:string)  [unwired: 9 in, 1 out]
                  n370 = call "To JSON Text.vim"("Anything"=w1270) -> ("<JSON>"=w1268:string)  [unwired: 9 in, 1 out]
                  n371 = case shown="True" w1258 {
                    tunnel: [string[] ["name", "description-en", "documentation-en", "dataType", "bitfield", "access", "min", "max", "scale"] ("Item Names") string[] ["name", "description-en", "documentation-en", "dataType", "bitfield", "access", "min", "max"] ("Item Names")] -> w1276
                    tunnel: [w1277 w1296] -> w1275
                    tunnel: w1274 -> [w1286 w1295]
                    tunnel: w1273 -> [w1285 w1294]
                    tunnel: w1272 -> [w1284 w1293]
                    tunnel: w1269 -> [w1280 w1292]
                    tunnel: w1268 -> [w1279 w1291]
                    tunnel: w1266 -> [w1283 w1290]
                    tunnel: w1264 -> [w1282 w1289]
                    tunnel: w1262 -> [w1281 w1288]
                    tunnel: w1257 -> [w1278 _]
                    frame False {
                      n372 = Build Array(w1286, w1285, w1284, w1283, w1282, w1281, w1280, w1279, w1278) -> (w1277:string[])
                    }
                    frame True {
                      n373 = Build Array(w1295, w1294, w1293, w1290, w1289, w1288, w1292, w1291) -> (w1296:string[])
                    }
                  }
                }
                frame False {
                  n374 = Equal?(x=w1300, y="NoScale") -> (x = y?=w1299:bool)
                  n375 = call "To JSON Text.vim"("Anything"=w1305) -> ("<JSON>"=w1304:string)  [unwired: 9 in, 1 out]
                  n376 = call "To JSON Text.vim"("Anything"=w1303) -> ("<JSON>"=w1302:string)  [unwired: 9 in, 1 out]
                  n377 = call "To JSON Text.vim"("Anything"="UInt32") -> ("<JSON>"=w1306:string)  [unwired: 9 in, 1 out]
                  n378 = call "To JSON Text.vim"("Anything"=w1300) -> ("<JSON>"=w1298:string)  [unwired: 9 in, 1 out]
                  n379 = case shown="True" w1299 {
                    tunnel: [string[] ["name", "description-en", "documentation-en", "dataType", "bitfield", "access", "scale"] ("Item Names") string[] ["name", "description-en", "documentation-en", "dataType", "bitfield", "access"] ("Item Names")] -> w1312
                    tunnel: [w1314 w1328] -> w1311
                    tunnel: w1310 -> [w1320 w1327]
                    tunnel: w1309 -> [w1319 w1326]
                    tunnel: w1308 -> [w1318 w1325]
                    tunnel: w1306 -> [w1317 w1324]
                    tunnel: w1304 -> [w1316 w1323]
                    tunnel: w1302 -> [w1315 w1322]
                    tunnel: w1298 -> [w1313 _]
                    frame False {
                      n380 = Build Array(w1320, w1319, w1318, w1317, w1316, w1315, w1313) -> (w1314:string[])
                    }
                    frame True {
                      n381 = Build Array(w1327, w1326, w1325, w1324, w1323, w1322) -> (w1328:string[])
                    }
                  }
                }
              }
            }
            frame "I32" {
              n382 = case shown="True" w1330 {
                tunnel: [w1359 w1395] -> w1339
                tunnel: w1338 -> [w1358 w1394]
                tunnel: [w1357 w1393] -> w1337
                tunnel: w1336 -> [w1356 w1392]
                tunnel: w1335 -> [w1355 w1391]
                tunnel: w1334 -> [w1348 w1388]
                tunnel: w1333 -> [w1347 w1387]
                tunnel: w1332 -> [w1344 _]
                tunnel: w1331 -> [w1342 w1383]
                frame True {
                  n383 = Unbundle By Name(w1344) -> ("Min(I32)"=w1354:i32, "Max(I32)"=w1353:i32)
                  n384 = call "To JSON Text.vim"("Anything"=w1347) -> ("<JSON>"=w1345:string)  [unwired: 9 in, 1 out]
                  n385 = call "To JSON Text.vim"("Anything"="Int32") -> ("<JSON>"=w1349:string)  [unwired: 9 in, 1 out]
                  n386 = call "To JSON Text.vim"("Anything"=w1348) -> ("<JSON>"=w1346:string)  [unwired: 9 in, 1 out]
                  n387 = Equal?(x=w1342, y="NoScale") -> (x = y?=w1340:bool)
                  n388 = call "To JSON Text.vim"("Anything"=w1353) -> ("<JSON>"=w1351:string)  [unwired: 9 in, 1 out]
                  n389 = call "To JSON Text.vim"("Anything"=w1354) -> ("<JSON>"=w1352:string)  [unwired: 9 in, 1 out]
                  n390 = call "To JSON Text.vim"("Anything"=w1342) -> ("<JSON>"=w1341:string)  [unwired: 9 in, 1 out]
                  n391 = case shown="False" w1340 {
                    tunnel: [string[] ["name", "description-en", "documentation-en", "dataType", "bitfield", "access", "min", "max", "scale"] ("Item Names") string[] ["name", "description-en", "documentation-en", "dataType", "bitfield", "access", "min", "max"] ("Item Names")] -> w1359
                    tunnel: w1358 -> [w1369 w1379]
                    tunnel: [w1368 w1378] -> w1357
                    tunnel: w1356 -> [w1367 w1377]
                    tunnel: w1355 -> [w1366 w1376]
                    tunnel: w1352 -> [w1362 w1375]
                    tunnel: w1351 -> [w1361 w1374]
                    tunnel: w1349 -> [w1365 w1373]
                    tunnel: w1346 -> [w1364 w1372]
                    tunnel: w1345 -> [w1363 w1371]
                    tunnel: w1341 -> [w1360 _]
                    frame False {
                      n392 = Build Array(w1369, w1367, w1366, w1365, w1364, w1363, w1362, w1361, w1360) -> (w1368:string[])
                    }
                    frame True {
                      n393 = Build Array(w1379, w1377, w1376, w1373, w1372, w1371, w1375, w1374) -> (w1378:string[])
                    }
                  }
                }
                frame False {
                  n394 = call "To JSON Text.vim"("Anything"=w1387) -> ("<JSON>"=w1385:string)  [unwired: 9 in, 1 out]
                  n395 = call "To JSON Text.vim"("Anything"="Int32") -> ("<JSON>"=w1389:string)  [unwired: 9 in, 1 out]
                  n396 = call "To JSON Text.vim"("Anything"=w1388) -> ("<JSON>"=w1386:string)  [unwired: 9 in, 1 out]
                  n397 = Equal?(x=w1383, y="NoScale") -> (x = y?=w1381:bool)
                  n398 = call "To JSON Text.vim"("Anything"=w1383) -> ("<JSON>"=w1382:string)  [unwired: 9 in, 1 out]
                  n399 = case shown="False" w1381 {
                    tunnel: [string[] ["name", "description-en", "documentation-en", "dataType", "bitfield", "access", "scale"] ("Item Names") string[] ["name", "description-en", "documentation-en", "dataType", "bitfield", "access"] ("Item Names")] -> w1395
                    tunnel: w1394 -> [w1403 w1411]
                    tunnel: [w1402 w1410] -> w1393
                    tunnel: w1392 -> [w1401 w1409]
                    tunnel: w1391 -> [w1400 w1408]
                    tunnel: w1389 -> [w1399 w1407]
                    tunnel: w1386 -> [w1398 w1406]
                    tunnel: w1385 -> [w1397 w1405]
                    tunnel: w1382 -> [w1396 _]
                    frame False {
                      n400 = Build Array(w1403, w1401, w1400, w1399, w1398, w1397, w1396) -> (w1402:string[])
                    }
                    frame True {
                      n401 = Build Array(w1411, w1409, w1408, w1407, w1406, w1405) -> (w1410:string[])
                    }
                  }
                }
              }
            }
            frame "Bool" {
              n402 = call "To JSON Text.vim"("Anything"="Bool") -> ("<JSON>"=w1417:string)  [unwired: 9 in, 1 out]
              n403 = call "To JSON Text.vim"("Anything"=w1416) -> ("<JSON>"=w1414:string)  [unwired: 9 in, 1 out]
              n404 = call "To JSON Text.vim"("Anything"=w1415) -> ("<JSON>"=w1413:string)  [unwired: 9 in, 1 out]
              n405 = Build Array(w1422, w1420, w1419, w1417, w1414, w1413) -> (w1421:string[])
            }
          }
        }
      }
      n406 = Unbundle By Name(w740) -> ("Selected Type and name.Selected Property Name"=w724:string, "Ref Cluster.Property tree"=w742:refnum<vi>)
      n407 = Unbundle By Name(w749) -> ("Physical Channel Index"=w746:i32, "Property Index"=w736:i32)
      n408 = Unbundle By Name(w743) -> ("NewPropertyParameter.Name"=w737:string)
      n409 = Number To Decimal String(number=w746) -> (decimal integer string=w750:string)  [unwired: 1 in]
      n410 = Index Array(array=w747, index=w746) -> (element=w727:string)
      n411 = call <vilib>:"Find Item.vi"("$Path or Item Name"="$.properties", "JSON"=w727) -> ("<JSON>"=w725:string)  [unwired: 6 in, 3 out]
      n412 = call <vilib>:"Get Array Elements.vi"("JSON"=w725) -> ("<JSON>"=w735:string[])  [unwired: 8 in, 2 out]
      n413 = call "ParserPropertyPath.vi"("Seleted Item Name"=w724) -> ("Physical channel"=w723:string)  [unwired: 7 in, 1 out]
      n414 = Concatenate Strings("$.physicalChannels[" ("$Path or Item Name"), w750, "].properties" ("string")) -> (w732:string)
      n415 = Concatenate Strings(w723, "/" ("regular expression"), w737) -> (w722:string)
      n416 = Bundle By Name(cluster=w740, "Selected Type and name.Selected Property Name"=w722) -> (w739:T2)
      n417 = Build Array(w722) -> (w741:string[])
      n418 = property class="Tree (strict)"(reference=w742, "Value"=w741) -> ()  [unwired: 1 in, 2 out]
      n419 = call "InsertIntoNewProperty.vi"("$Path or Item Name"=w732, "JSON Items"=w733, "JSON In"=w731, "error in (no error)"=w728, "Item Names"=w734, "index"=w736, "Input array"=w735) -> ("error out"=w729:errorcluster, "<JSON>"=w730:string)  [unwired: 3 in]
    }
  }
  "Data Out" <- w11
  "JSON Text Out" <- w10
  "error out" <- w9
